vi "VIH UI - Property Page - File.vi"() -> ()   [LabVIEW 2014]
doc: "::: VI Helpeks :::\nCopyright (c) 2000-2026 Konstantin Shifershteyn. All rights reserved."
uses:
  _VIH HelpGen.llb/VIH HelpGen Typedef - Enum - Default,Enable,Disable.ctl
  _VIH HelpGen.llb/VIH HelpGen Typedef - Enum - Description Mode.ctl
  _VIH UI Controls.llb/VIH UI Control - Button - Insert HREF.ctl
  _VIH UI Controls.llb/VIH UI Control - Button - Insert Bold.ctl
  _VIH UI Controls.llb/VIH UI Control - Button - Insert Italic.ctl
  _VIH UI Controls.llb/VIH UI Control - Button - Insert Underline.ctl
  _VIH Project Manager.llb/VIH Project Tree Typedef - Tree Refnum.ctl
  VIH UI Typedef - Property Page ExtCommand.ctl
  <vilib>/Utility/miscctls.llb/LVPositionTypeDef.ctl
  <vilib>/Utility/miscctls.llb/LVPointTypeDef.ctl
  <vilib>/Utility/miscctls.llb/LVRowAndColumnUnsignedTypeDef.ctl
  <vilib>/Utility/miscctls.llb/LVSelectionTypeDef.ctl
  _VIH HelpGen - Palette.llb/VIH HelpGen Typedef - Palette - Item Type Enum.ctl
  _VIH Support Library.llb/VIH Utility - APP - Is Value Changed (STR).vi
  _VIH Support Library.llb/VIH Utility - APP - Is Value Changed (BOOL).vi
panel:
  out "CategoryTitle":string
  in  "%UPDATE":bool
  in  "%STOP":bool
  in  "Category List":i32(listbox)
  in  "TreeRef":T1
  in  "Tab Control":enum32{"0", "1", "2", "3", "4", "5", "6", "7"}(tab) caption="File Rule"
  out "PI_AddInfo":string caption="Additional Information"
  out "PI_Email":string caption="Contact E-mail"
  out "PI_Website":string caption="Website"
  out "PI_Version":string caption="Version"
  out "PI_Copyright":string caption="Legal Copyright"
  out "PI_Company":string caption="Company Name"
  out "PI_Author":string caption="Author Name"
  out "PI_Product":string caption="Product Name"
  in  "ProductInfoText":string caption="Product Info section"
  in  "ProductInfoMode":u16(ring) caption="Product Info mode" items=["Default", "Custom", "Disable"]
  out "Out File Path":path caption="Output File Path"
  in  "Out File Name":string caption="Output File Name"
  in  "Custom_OutFile":i16(ring) caption="Default/Custom selector" items=["Default", "Custom"]
  in  "BuildHelp":T2 caption="Build help for this file"
  out "File Name":string
  in  "Comments":string
  in  "Custom_JS Dir":i16(ring) caption="Default/Custom selector" items=["Default", "Custom"]
  in  "Dst_JS Dir":path caption="Subfolder to save JavaScript files"
  in  "Custom_CSS Dir":i16(ring) caption="Default/Custom selector" items=["Default", "Custom"]
  in  "Dst_CSS Dir":path caption="Subfolder to save CSS files"
  in  "Custom_Image Dir":i16(ring) caption="Default/Custom selector" items=["Default", "Custom"]
  in  "Dst_Image Dir":path caption="Subfolder to save image files"
  in  "Custom_HTML Dir":i16(ring) caption="Default/Custom selector" items=["Default", "Custom"]
  in  "Dst_HTML Dir":path caption="Subfolder to save HTML files"
  out "Build Root Dir":path caption="Build Root Folder"
  in  "Src_Template":path caption="Help Template File"
  in  "Custom_Template":i16(ring) caption="Default/Custom selector" items=["Default", "Custom"]
  out "JS File":path caption="JS File Path"
  in  "JS List":i32[](listbox) caption="JavaScript Files"
  in  "%JS List_Add":bool caption="Add JavaScript File"
  in  "%JS List_Remove":bool caption="Remove JavaScript File"
  in  "Override_JS Files":bool caption="Override default JS file set"
  out "CSS File":path caption="CSS File Path"
  in  "CSS List":i32[](listbox) caption="CSS Files"
  in  "%CSS List_Add":bool caption="Add CSS File"
  in  "%CSS List_Remove":bool caption="Remove CSS File"
  in  "Override_CSS Files":bool caption="Override default CSS file set"
  in  "%VIDetails_Insert_<I>":T3 caption="Format as Italic"
  in  "%VIDetails_Insert_<U>":T4 caption="Format as Underline"
  in  "%VIDetails_Insert_<B>":T5 caption="Format as Bold"
  in  "%VIDetails_Insert_HREF":T6 caption="Insert Reference"
  in  "VIDetails":string caption="Details section"
  in  "VIDetailsMode":T7 caption="Details section mode"
  in  "%VIDscr_Insert_<I>":T3 caption="Format as Italic"
  in  "%VIDscr_Insert_<U>":T4 caption="Format as Underline"
  in  "%VIDscr_Insert_<B>":T5 caption="Format as Bold"
  in  "%VIDscr_Insert_HREF":T6 caption="Insert Reference"
  in  "VIDescription":string caption="Description"
  in  "MenuItemIcons":T2 caption="Generate Palette Item Icons"
  in  "VIDscrMode":T7 caption="Description mode"
  in  "Ctl_EnumValues":T2 caption="Build list of Enum and Ring values"
  in  "Ctl_ClustMembers":T2 caption="Expand cluster members"
  in  "Ctl_DscrMode":T7 caption="VI Controls/Terminals description mode"
  in  "%CtrlRule_Insert_<I>":T3 caption="Format as Italic"
  in  "%CtrlRule_Insert_<U>":T4 caption="Format as Underline"
  in  "%CtrlRule_Insert_<B>":T5 caption="Format as Bold"
  in  "%CtrlRule_Insert_HREF":T6 caption="Insert Reference"
  in  "CtrlRule_Description":string caption="Description"
  in  "CtrlRule_CustomName":string caption="Custom Control Name"
  in  "CtrlRule_DscrMode":T7 caption="Description mode"
  in  "CtrlRule_CustomRule":bool caption="Enable custom rule"
  in  "CtrlRule_CtrlID":string caption="Control Identifier"
  in  "%CtrlRule_Edit_Enum":bool caption="Edit Enumerated Values Description"
  in  "CtrlRule_EnumValues":T2 caption="Enum and Ring values"
  in  "CtrlRule_ClustMembers":T2 caption="Cluster members"
  in  "%CtrlRule_Copy":bool caption="Copy"
  in  "%CtrlRule_Paste":bool caption="Paste"
  in  "%CtrlRule_Import":bool caption="Import VI Terminal Controls"
  in  "CtrlRule List":i32[](listbox) caption="Control List"
  in  "%CtrlRule_Remove":bool caption="Remove"
  in  "%CtrlRule_Add":bool caption="Add"
  in  "Override_Ctl Rules":bool caption="Override default Control Rules definition"
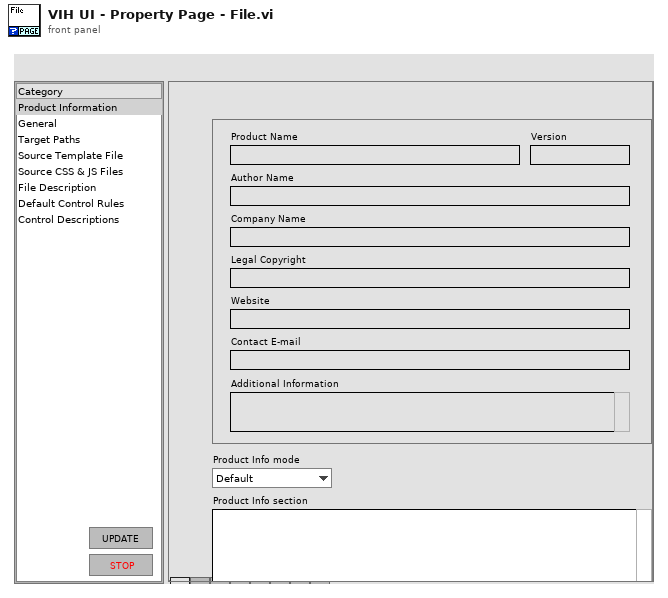
[diagram p1: front panel]
types:
  T1 = typedef "VIH Project Tree Typedef - Tree Refnum.ctl" = refnum<vi>
  T2 = typedef "VIH HelpGen Typedef - Enum - Default,Enable,Disable.ctl" = enum16{"Default", "Enable", "Disable"}
  T3 = typedef "VIH UI Control - Button - Insert Italic.ctl" = bool
  T4 = typedef "VIH UI Control - Button - Insert Underline.ctl" = bool
  T5 = typedef "VIH UI Control - Button - Insert Bold.ctl" = bool
  T6 = typedef "VIH UI Control - Button - Insert HREF.ctl" = bool
  T7 = typedef "VIH HelpGen Typedef - Enum - Description Mode.ctl" = enum16{"Default", "Description", "Description1", "Description2", "Custom", "None"}
  T8 = typedef "VIH UI Typedef - Property Page ExtCommand.ctl" = cluster{"Action":string, "Project Tree":T1, "Params":string[]}
  T9 = enum16{"Open", "Close", "Update", "Set Category"}
  T10 = enum32{"Invalid", "Standard", "Closed", "Hidden", "Minimized", "Maximized"}
  T11 = enum8{"Enabled", "Disabled", "Disabled and Grayed Out"}
  T12 = typedef "LVSelectionTypeDef.ctl" = cluster{"Selection Start":u32, "Selection End":u32}
  T13 = enum16{"get", "get all", "set", "Init", "delete", "rename"}
  T14 = typedef "eventvkey.ctl" = enum16{"ASCII", "Enter", "Return", "Shift", "Ctrl", "Alt", "Cmd", "Opt", "Caps", "NumLock", "Clear", "Break", "Up", "Down", "Left", "Right", "Insert", "Delete", "Home", "End", "PageUp", "PageDown", "Escape", "Help", "Pause", "ScrollLock", "F1", "F2", "F3", "F4", "F5", "F6", "F7", "F8", "F9", "F10", "F11", "F12", "F13", "F14", "F15", "F16", "F17", "F18", "F19", "F20", "F21", "F22", "F23", "F24", "Play", "VolumeUp", "VolumeDown", "Mute", "Two Byte Char"}
  T15 = cluster{"Shift":bool, "Ctrl":bool, "Alt":bool, "Cmd":bool, "Opt":bool}
  T16 = typedef "VIH HelpGen Typedef - Cluster - Group Rule.ctl" = cluster{"Source Root Dir":path, "Build Root Dir":path, "BuildHelp":T2, "Source Paths":T17, "Target Paths":T18, "VIDscrMode":T7, "MenuDscrMode":T7, "MenuItemIcons":T2, "Control Rules":T19[], "Flags":T21, "Ctl_DscrMode":T7, "Ctl_ClustMembers":T2, "Ctl_EnumValues":T2, "%Comments":string, "PVIIDscrMode":T7, "VIDetailsMode":T7, "ProductInfoMode":T2, "ProductInfoText":string}
  T17 = typedef "VIH HelpGen Typedef - Cluster - Group Rule - Source Paths.ctl" = cluster{"CSS Files":path[], "JS Files":path[], "VI Template":path, "Menu Template":path, "PolyVI Template":path}
  T18 = typedef "VIH HelpGen Typedef - Cluster - Group Rule - Target Paths.ctl" = cluster{"HTML Dir":path, "Image Dir":path, "CSS Dir":path, "JS Dir":path}
  T19 = typedef "VIH HelpGen Typedef - Cluster - Control Rule.ctl" = cluster{"CtrlID":string, "CustomRule":bool, "DscrMode":T7, "Description":string, "ClusterMembers":T2, "EnumValues":T2, "EnumValDscr":T20[], "CustomName":string}
  T20 = typedef "VIH HelpGen Typedef - Cluster - Enum Value Info.ctl" = cluster{"Value":ext, "String":string, "Description":string}
  T21 = typedef "VIH HelpGen Typedef - Cluster - Group Rule - Flags.ctl" = cluster{"Override CSS Files":bool, "Override JS Files":bool, "Override Ctl Rules":bool}
  T22 = typedef "LVPoint32TypeDef.ctl" = cluster{"Horizontal":i32, "Vertical":i32}
  T23 = typedef "LVRowAndColumnTypeDef.ctl" = cluster{"Row":i32, "Column":i32}
  T24 = typedef "lveventtype.ctl" = enum32{"Null", "Timeout", "Annotation Menu Selection", "Annotation Menu Selection?", "App Instance Close", "App Instance Close?", "Autoscale Range Change", "Bookmark Info Change", "Cell Edit", "Cell Edit?", "Cursor Grab", "Cursor Grab?", "Cursor Menu Selection", "Cursor Menu Selection?", "Cursor Move", "Cursor Release", "Data Change", "Direction Change", "Display State Change", "Drag Ended", "Drag Enter", "Drag Leave", "Drag Over", "Drag Source Update", "Drag Starting", "Drag Starting?", "Drop", "Exec State Change", "Key Down", "Key Down?", "Key Repeat", "Key Repeat?", "Key Up", "Listbox Double Click", "Menu Activation?", "Menu Selection (App)", "Menu Selection? (App)", "Menu Selection (User)", "Mouse Down", "Mouse Down?", "Mouse Enter", "Mouse Leave", "Mouse Move", "Mouse Up", "Mouse Wheel", "NI Security User Change (App)", "Pane Size", "Panel Close", "Panel Close?", "Panel Resize", "Plot Attribute Change", "Scale Range Change", "Shortcut Menu Activation?", "Shortcut Menu Selection (App)", "Shortcut Menu Selection? (App)", "Shortcut Menu Selection (User)", "Tree Double Click", "Tree Drag", "Tree Drag?", "Tree Drop", "Tree Drop?", "Tree Item Close", "Tree Item Close?", "Tree Item Open", "Tree Item Open?", "User Event", "Value Change"}
  T25 = typedef "LVPointTypeDef.ctl" = cluster{"Horizontal":i16, "Vertical":i16}
  T26 = typedef "LVPositionTypeDef.ctl" = cluster{"Left":i32, "Top":i32}
  T27 = typedef "LVRowAndColumnUnsignedTypeDef.ctl" = cluster{"Row":u32, "Column":u32}
  T28 = typedef "VIH Project Tree Typedef - Tree Item Type.ctl" = enum32{"<Invalid>", "Project", "Proj Files", "Proj Rules", "File Group", "Rule Group", "Any File", "LV Func", ".mnu", ".mnu (dyn)", ".vi", ".vi (dyn)", ".vit", ".vit (dyn)", ".ctl", ".ctl (dyn)", ".ctt", ".ctt (dyn)", "polyVI", "polyVI (dyn)", "expVI", "expVI (dyn)", "HTML", "PolyVI Inst"}
  T29 = typedef "VIH HelpGen Typedef - Cluster - File Rule.ctl" = cluster{"OutName":string, "BuildHelp":T2, "Source Paths":T30, "Target Paths":T31, "DscrMode":T7, "Description":string, "Control Rules":T19[], "Flags":T21, "Ctl_DscrMode":T7, "Ctl_ClustMembers":T2, "Ctl_EnumValues":T2, "MenuItemIcons":T2, "%Comments":string, "DetailsMode":T7, "DetailsText":string, "ProductInfoMode":T2, "ProductInfoText":string}
  T30 = typedef "VIH HelpGen Typedef - Cluster - File Rule - Source Paths.ctl" = cluster{"CSS Files":path[], "JS Files":path[], "Html Template":path}
  T31 = typedef "VIH HelpGen Typedef - Cluster - File Rule - Target Paths.ctl" = cluster{"HTML Dir":path, "Image Dir":path, "CSS Dir":path, "JS Dir":path}
  T32 = cluster{"Array out":string[], "Item Rule out":T29}
  T33 = typedef "VIH HelpGen Typedef - Palette - Item Type Enum.ctl" = enum32{"<Invalid>", "<unknown>", "VI", "Menu", "LV Func", "Express VI", "Poly VI", "CTL", "HTML"}
  T34 = typedef "VIH HelpGen Typedef - Product Info Cluster.ctl" = cluster{"ProductName":string, "Version":string, "Author":string, "Company":string, "Copyright":string, "Website":string, "Email":string, "AddInfo":string}
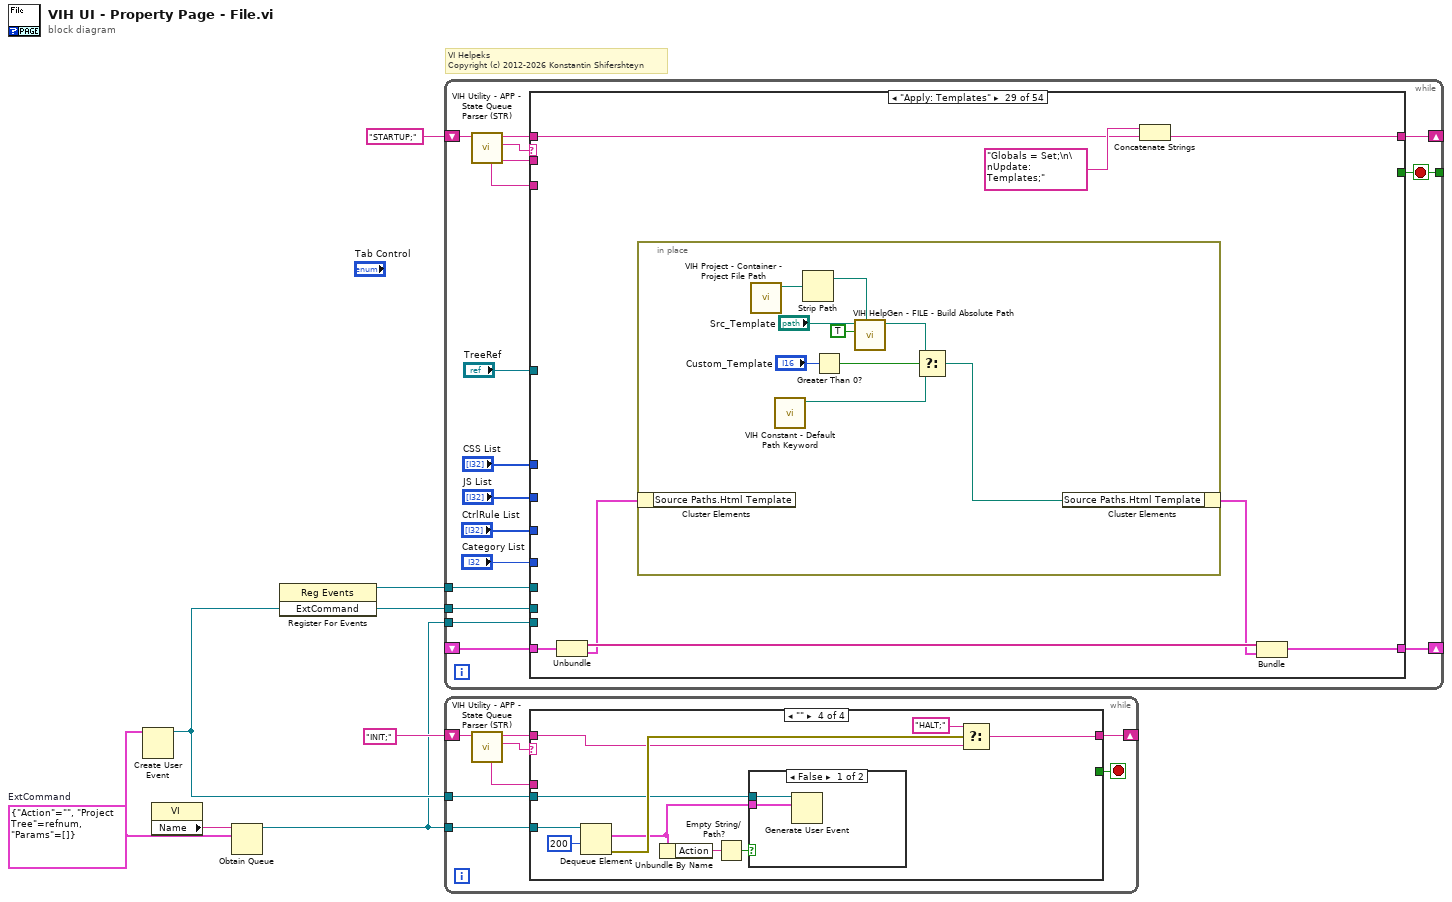
[diagram p0: block diagram]
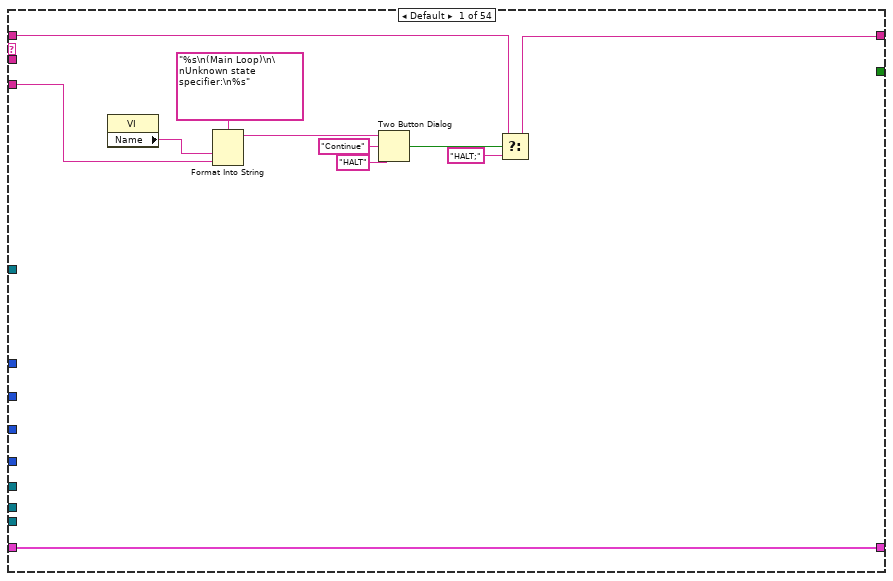
[diagram p2: hidden frame]
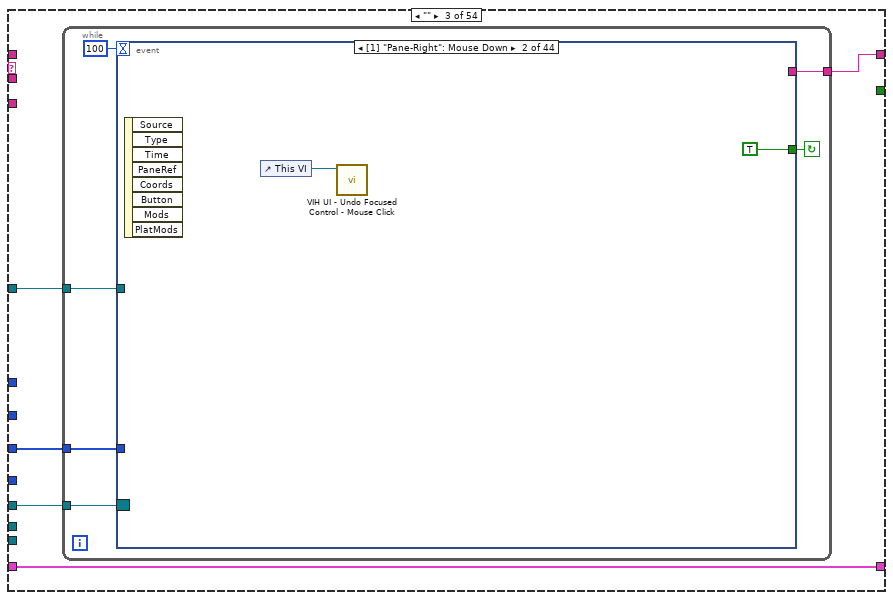
[diagram p4: hidden frame]
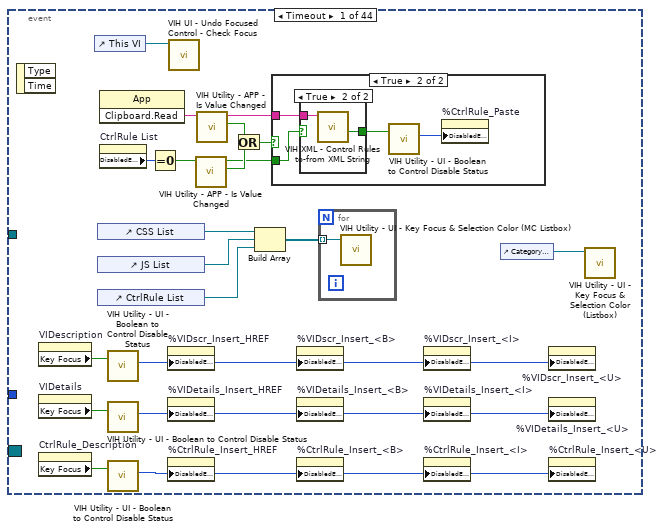
[diagram p5: hidden frame]
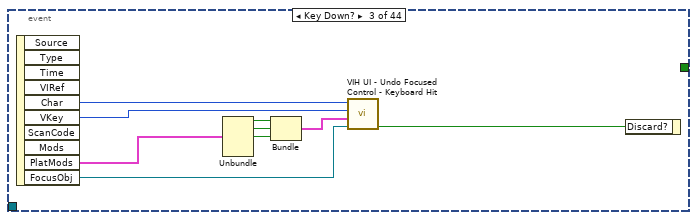
[diagram p8: hidden frame]
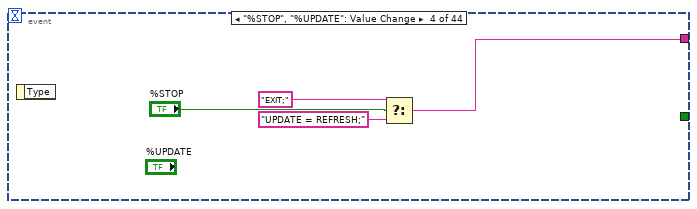
[diagram p9: hidden frame]
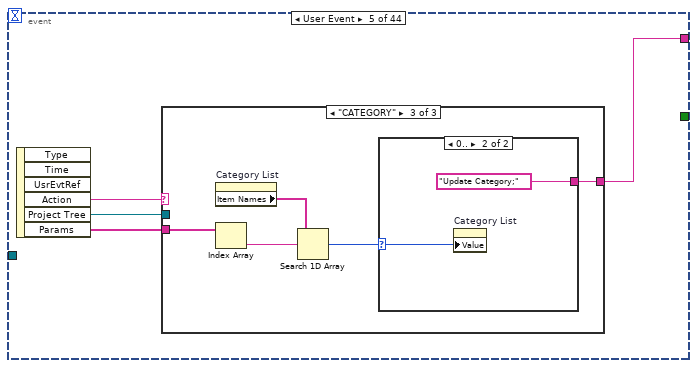
[diagram p10: hidden frame]
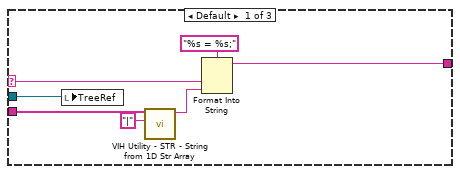
[diagram p11: hidden frame]
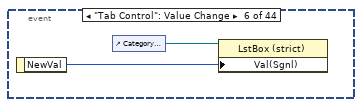
[diagram p14: hidden frame]
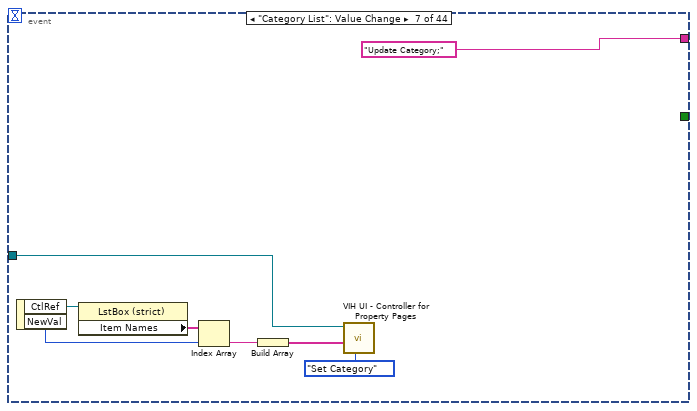
[diagram p15: hidden frame]
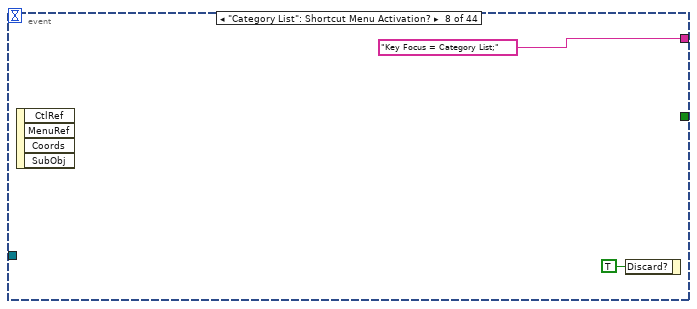
[diagram p16: hidden frame]
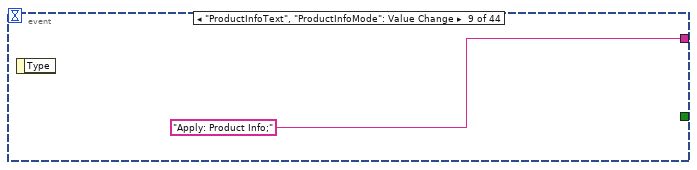
[diagram p17: hidden frame]
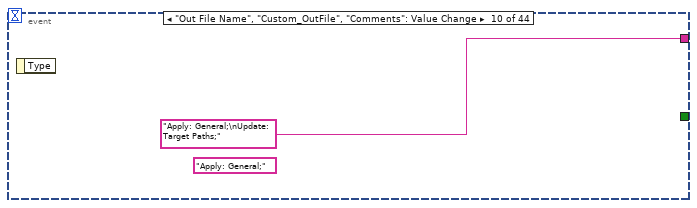
[diagram p18: hidden frame]
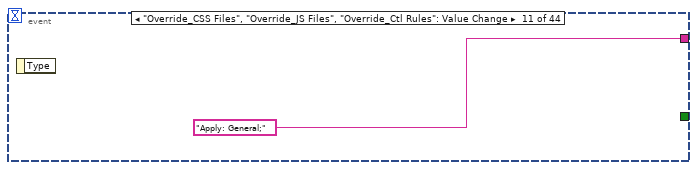
[diagram p19: hidden frame]
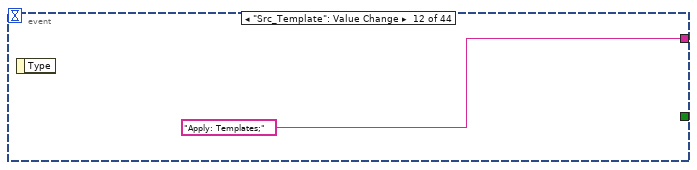
[diagram p20: hidden frame]
diagram:
  w1 = T8 {"Action"="", "Project Tree"=refnum, "Params"=[]}  # ExtCommand
  # "VI Helpeks\nCopyright (c) 2012-2026 Konstantin Shifershteyn"
  n1 = Create User Event(user event datatype=w1) -> (user event=w3:refnum<user-event>)  [unwired: 1 in, 1 out]
  n2 = property class="VI"() -> ("Name"=w6:string)  [unwired: 2 in, 2 out]
  n3 = Obtain Queue(name (unnamed)=w6, element data type=w1) -> (queue out=w2:refnum<queue>)  [unwired: 3 in, 2 out]
  n4 = register-events(w3) -> (reference out=w5:refnum<event-registration>)  [unwired: 2 in, 1 out]
  n5 = while {
    shift-right: [w21] -> _
    shift-left: "STARTUP;" -> [w24]
    tunnel: [w19] -> _
    tunnel: w5 -> [w18]
    tunnel: w3 -> [w17]
    tunnel: w2 -> [w16]
    shift-right: [w13] -> _
    shift-left: _ -> [w12]
    stop <- w19 stop-if-true
    n6 = call "VIH Utility - APP - State Queue Parser (STR).vi"("input queue"=w24) -> ("state parameters"=w15:string, "state"=w23:string, "remained queue"=w20:string, "complete state specifier"=w22:string)  [unwired: 5 in]
    n7 = case shown="\"Apply: Templates\"" w23 {
      tunnel: w22 -> [w31 _ _ _ _ _ _ _ _ w469 _ _ _ _ _ _ _ _ _ _ _ _ _ _ _ _ _ _ _ _ _ _ _ _ _ _ _ _ _ _ _ _ _ _ _ _ _ _ _ _ _ _ _ _]
      tunnel: [w26 w36 w41 "INIT;\nUPDATE;" w391 "HALT;" w417 w420 w444 w471 w497 w521 w525 w541 w547 w557 w620 w693 w716 w772 w803 w815 w878 w901 w921 w922 w935 w954 w979 w996 w1013 w1030 w1077 w1105 w1148 w1155 w1179 w1195 w1231 w1253 w1280 w1288 w1306 w1318 w1344 w1368 w1383 w1391 w1409 w1421 w1447 w1471 w1486 w1488] -> w21
      tunnel: w20 -> [w27 w36 _ _ w391 _ w417 w420 w445 w471 w497 w521 w525 w541 w547 w557 w620 w693 w716 w772 w803 w843 w878 w901 w921 w923 w941 w955 w980 w997 w1013 w1030 w1082 w1106 w1148 w1160 w1184 w1202 w1236 w1260 w1280 w1288 w1306 w1322 w1349 w1373 w1383 w1391 w1409 w1425 w1452 w1476 w1486 w1488]
      tunnel: [_ _ _ _ _ _ TRUE _ _ _ _ _ _ _ _ _ _ _ _ _ _ _ _ _ _ _ _ _ _ _ _ _ _ _ _ _ _ _ _ _ _ _ _ _ _ _ _ _ _ _ _ _ _ _] -> w19
      tunnel: w18 -> [_ _ w42 _ _ _ w416 _ _ _ _ _ _ _ _ _ _ _ _ _ _ _ _ _ _ _ _ _ _ _ _ _ _ _ _ _ _ _ _ _ _ _ _ _ _ _ _ _ _ _ _ _ _ _]
      tunnel: w17 -> [_ _ _ _ _ _ w415 _ _ _ _ _ _ _ _ _ _ _ _ _ _ _ _ _ _ _ _ _ _ _ _ _ _ _ _ _ _ _ _ _ _ _ _ _ _ _ _ _ _ _ _ _ _ _]
      tunnel: w16 -> [_ _ _ _ _ _ w413 _ _ _ _ _ _ _ _ _ _ _ _ _ _ _ _ _ _ _ _ _ _ _ _ _ _ _ _ _ _ _ _ _ _ _ _ _ _ _ _ _ _ _ _ _ _ _]
      tunnel: w15 -> [_ _ _ _ _ _ _ _ w431 w470 _ w519 w523 _ _ _ _ _ _ w761 w794 _ _ w888 _ _ _ _ _ _ _ w1014 _ w1100 _ _ _ w1193 w1228 w1251 _ _ _ _ _ _ _ _ _ _ _ _ _ _]
      tunnel: "Category List" -> [_ _ _ _ _ _ _ _ _ _ w494 _ _ _ _ _ _ _ _ _ _ _ _ _ _ _ _ _ _ _ _ _ _ _ _ _ _ _ _ _ _ _ _ _ _ _ _ _ _ _ _ _ _ _]
      tunnel: [w25 w37 w40 w363 w390 w398 w411 w419 w442 w473 w491 w520 w524 w540 w546 w574 w619 w692 w715 w771 w802 w842 w877 w900 w920 w927 w938 w959 w984 w1001 w1012 w1029 w1078 w1104 w1145 w1156 w1180 w1197 w1232 w1255 w1279 w1286 w1305 w1319 w1345 w1369 w1382 w1389 w1408 w1422 w1448 w1472 w1485 w1487] -> w13
      tunnel: w12 -> [w25 w37 w40 w363 w390 w398 w411 w419 w441 w472 w491 w520 w524 w540 w546 w574 w619 w692 w715 w771 w802 w842 w877 w900 w920 w929 w940 w961 w986 w1003 w1012 w1029 w1079 w1095 w1145 w1157 w1181 w1198 w1233 w1256 w1279 w1286 w1305 w1320 w1346 w1370 w1382 w1389 w1408 w1423 w1449 w1473 w1485 w1487]
      tunnel: "CtrlRule List" -> [_ _ w39 _ _ _ _ _ _ _ _ _ _ _ _ _ _ _ _ _ _ _ _ w890 _ _ _ _ _ _ _ w1021 w1071 w1098 w1146 w1153 _ _ _ _ _ _ _ _ _ _ _ _ _ _ _ _ _ _]
      tunnel: "CSS List" -> [_ _ _ _ _ _ _ _ _ _ _ _ _ _ _ _ _ _ _ w763 _ _ _ _ _ _ _ _ _ _ _ _ _ _ _ _ _ _ _ _ _ w1285 _ w1310 w1342 _ _ _ _ _ _ _ _ _]
      tunnel: "JS List" -> [_ _ _ _ _ _ _ _ _ _ _ _ _ _ _ _ _ _ _ _ w793 _ _ _ _ _ _ _ _ _ _ _ _ _ _ _ _ _ _ _ _ _ _ _ _ _ _ w1387 _ w1411 w1445 _ _ _]
      tunnel: "TreeRef" -> [_ _ w38 _ _ _ _ _ _ _ _ _ _ _ _ _ _ w656 w707 _ _ _ _ _ _ _ _ _ _ _ _ _ _ w1096 _ _ _ _ _ w1250 _ _ _ _ _ _ _ _ _ _ _ _ _ _]
      frame Default {
        n8 = property class="VI"() -> ("Name"=w30:string)  [unwired: 2 in, 2 out]
        n9 = Format Into String(format string="%s\n(Main Loop)\n\nUnknown state specifier:\n%s", w30, w31) -> (resulting string=w34:string)  [unwired: 2 in, 1 out]
        n10 = Two Button Dialog(message=w34, 1:"HALT" ("F button name (\"Cancel\")"), 2:"Continue" ("T button name (\"OK\")")) -> (T button?=w28:bool)
        n11 = Select(t=w27, s=w28, f="HALT;") -> (s? t:f=w26:string)
      }
      frame "#" {
      }
      frame "" {
        n12 = while {
          tunnel: w42 -> [w47]
          tunnel: [w46] -> w41
          tunnel: w39 -> [w45]
          tunnel: w38 -> [w44]
          stop <- w43 continue-if-true
          n13 = event shown="[1] \"Pane-Right\": Mouse Down" {
            selector: w47 -> [_ _ _ _ _ _ _ _ _ _ _ _ _ _ _ _ _ _ _ _ _ _ _ _ _ _ _ _ _ _ _ _ _ _ _ _ _ _ _ _ _ _ _ _]
            dyn-events: _ -> [_ _ _ _ _ _ _ _ _ _ _ _ _ _ _ _ _ _ _ _ _ _ _ _ _ _ _ _ _ _ _ _ _ _ _ _ _ _ _ _ _ _ _ _]
            timeout: 100 -> [_ _ _ _ _ _ _ _ _ _ _ _ _ _ _ _ _ _ _ _ _ _ _ _ _ _ _ _ _ _ _ _ _ _ _ _ _ _ _ _ _ _ _ _]
            tunnel: [_ _ _ w89 w95 _ "Update Category;" ("string") "Key Focus = Category List;" ("output string") "Apply: Product Info;" ("string") "Apply: General;\nUpdate: Target Paths;" ("string") "Apply: General;" ("string") "Apply: Templates;" ("string") "Apply: Templates;" ("string") "Apply: Target Paths;" ("string") "Apply: Target Paths;" ("string") "Apply: Item Rules;" ("string") "Apply: Item Rules;" ("string") "CtrlRule: Update Controls = INIT;" ("string") w171 w185 w200 w215 "Key Focus = CtrlRule List;" ("output string") w219 w229 w242 w248 "CSS List: Update Controls;" w254 "Key Focus = CSS List;" ("output string") w258 "JS List: Update Controls;" w267 "Key Focus = JS List;" ("output string") w271 _ _ _ _ _ _ _ _ _] -> w46
            tunnel: w45 -> [_ _ _ _ _ _ _ _ _ _ _ _ _ _ _ _ _ _ _ w183 _ _ _ _ _ w235 w245 _ _ _ _ _ _ _ _ _ _ _ _ _ _ _ _ _]
            tunnel: w44 -> [_ _ _ _ _ _ w112 _ _ _ _ _ _ _ _ _ _ _ _ _ _ _ _ _ _ _ _ _ _ _ _ _ _ _ _ w284 w297 w309 w318 w322 w327 w331 w336 w340]
            tunnel: [_ TRUE _ _ _ _ _ _ _ _ _ _ _ _ _ _ _ _ _ _ _ _ _ _ _ _ _ _ _ _ _ _ _ _ _ _ _ _ _ _ _ _ _ _] -> w43
            event Timeout {
              n14 = event-data() -> ()  [unwired: 1 in, 2 out]
              n15 = property on="VIDescription" class="Str"() -> ("Key Focus"=w59:bool)  [unwired: 2 in, 2 out]
              n16 = property on="VIDetails" class="Str"() -> ("Key Focus"=w51:bool)  [unwired: 2 in, 2 out]
              n17 = property on="CtrlRule_Description" class="Str"() -> ("Key Focus"=w61:bool)  [unwired: 2 in, 2 out]
              n18 = control-ref of="This VI"() -> (w49:refnum<vi>)
              n19 = control-ref of="CSS List"() -> (w66:refnum<vi>)
              n20 = control-ref of="JS List"() -> (w65:refnum<vi>)
              n21 = control-ref of="CtrlRule List"() -> (w64:refnum<vi>)
              n22 = invoke class="App" method="Clipboard.Read"() -> ("Read Clipbrd"=w63:string)  [unwired: 3 in, 2 out]
              n23 = property on="CtrlRule List" class="MCListbox (strict)"() -> ("DisabledEnum"=w57:T11)  [unwired: 2 in, 2 out]
              n24 = call "VIH Utility - UI - Boolean to Control Disable Status.vi"("Status in"=w59) -> ("Control Disable if False"=w58:u8)  [unwired: 3 in, 1 out]
              n25 = call "VIH Utility - UI - Boolean to Control Disable Status.vi"("Status in"=w51) -> ("Control Disable if False"=w50:u8)  [unwired: 3 in, 1 out]
              n26 = call "VIH Utility - UI - Boolean to Control Disable Status.vi"("Status in"=w61) -> ("Control Disable if False"=w60:u8)  [unwired: 3 in, 1 out]
              n27 = Equal To 0?(x=w57) -> (x = 0?=w56:bool)
              n28 = property on="%VIDscr_Insert_HREF" class="Bool"("DisabledEnum"=w58) -> ()  [unwired: 2 in, 2 out]
              n29 = property on="%VIDetails_Insert_HREF" class="Bool"("DisabledEnum"=w50) -> ()  [unwired: 2 in, 2 out]
              n30 = property on="%CtrlRule_Insert_HREF" class="Bool"("DisabledEnum"=w60) -> ()  [unwired: 2 in, 2 out]
              n31 = call "VIH UI - Undo Focused Control - Check Focus.vi"("VI Refnum"=w49) -> ()  [unwired: 10 in, 1 out]
              n32 = call-poly "VIH Utility - APP - Is Value Changed.vi"("Value"=w56) -> ("Changed"=w54:bool, "dup Value"=w52:bool)  [unwired: 5 in]
              n33 = call-poly "VIH Utility - APP - Is Value Changed.vi"("Value"=w63) -> ("Changed"=w55:bool, "dup Value"=w62:string)  [unwired: 5 in]
              n34 = Or(x=w55, y=w54) -> (x .or. y?=w53:bool)
              n35 = Build Array(w66, w65, w64) -> (w68:refnum<vi>[])
              n36 = case shown="True" w53 {
                tunnel: w62 -> [_ w70]
                tunnel: w52 -> [_ w69]
                frame False {
                }
                frame True {
                  n37 = case shown="True" w69 {
                    selector: w69 -> [w73 _]
                    tunnel: [w73 w75] -> w72
                    tunnel: w70 -> [_ w74]
                    frame False {
                    }
                    frame True {
                      n38 = call "VIH XML - Control Rules to-from XML String.vi"("XML in"=w74) -> ("available"=w75:bool)  [unwired: 7 in, 3 out]
                    }
                  }
                  n39 = call "VIH Utility - UI - Boolean to Control Disable Status.vi"("Status in"=w72) -> ("Control Disable if False"=w71:u8)  [unwired: 3 in, 1 out]
                  n40 = property on="%CtrlRule_Paste" class="Bool"("DisabledEnum"=w71) -> ()  [unwired: 2 in, 2 out]
                }
              }
              n41 = property on="%VIDscr_Insert_<B>" class="Bool"("DisabledEnum"=w58) -> ()  [unwired: 2 in, 2 out]
              n42 = property on="%VIDetails_Insert_<B>" class="Bool"("DisabledEnum"=w50) -> ()  [unwired: 2 in, 2 out]
              n43 = property on="%CtrlRule_Insert_<B>" class="Bool"("DisabledEnum"=w60) -> ()  [unwired: 2 in, 2 out]
              n44 = for {
                tunnel: w68 -> [w76] mode=indexing
                n45 = call "VIH Utility - UI - Key Focus & Selection Color (MC Listbox).vi"("MCListbox Refnum"=w76) -> ()  [unwired: 8 in, 3 out]
              }
              n46 = property on="%VIDscr_Insert_<I>" class="Bool"("DisabledEnum"=w58) -> ()  [unwired: 2 in, 2 out]
              n47 = property on="%VIDetails_Insert_<I>" class="Bool"("DisabledEnum"=w50) -> ()  [unwired: 2 in, 2 out]
              n48 = property on="%CtrlRule_Insert_<I>" class="Bool"("DisabledEnum"=w60) -> ()  [unwired: 2 in, 2 out]
              n49 = control-ref of="Category List"() -> (w67:refnum<vi>)
              n50 = property on="%VIDscr_Insert_<U>" class="Bool"("DisabledEnum"=w58) -> ()  [unwired: 2 in, 2 out]
              n51 = property on="%VIDetails_Insert_<U>" class="Bool"("DisabledEnum"=w50) -> ()  [unwired: 2 in, 2 out]
              n52 = property on="%CtrlRule_Insert_<U>" class="Bool"("DisabledEnum"=w60) -> ()  [unwired: 2 in, 2 out]
              n53 = call "VIH Utility - UI - Key Focus & Selection Color (Listbox).vi"("LstBox Refnum"=w67) -> ()  [unwired: 8 in, 3 out]
            }
            event Mouse Down {
              n54 = event-data() -> ()  [unwired: 1 in, 8 out]
              n55 = control-ref of="This VI"() -> (w78:refnum<vi>)
              n56 = call "VIH UI - Undo Focused Control - Mouse Click.vi"("VI Refnum"=w78) -> ()  [unwired: 9 in, 2 out]
            }
            event Key Down? {
              n57 = event-data() -> ("Char"=w83:i16, "VKey"=w82:T14, "PlatMods"=w81:T15, "FocusObj"=w80:refnum<vi>)  [unwired: 1 in, 6 out]
              n58 = Unbundle(w81) -> ("Shift"=w84:bool, "Ctrl"=w85:bool, "Alt"=w86:bool)  [unwired: 2 out]
              n59 = Bundle("Shift"=w84, "Ctrl"=w85, "Alt"=w86) -> (w87:cluster{"Shift":bool, "Ctrl":bool, "Alt":bool})  [unwired: 1 in]
              n60 = call "VIH UI - Undo Focused Control - Keyboard Hit.vi"("FocusObj"=w80, "PlatMods"=w87, "VKey"=w82, "Char"=w83) -> ("Discard"=w79:bool)  [unwired: 7 in]
              n61 = event-data("Discard?"=w79) -> ()  [unwired: 1 in, 1 out]
            }
            event "%STOP", "%UPDATE": Value Change {
              n62 = event-data() -> ()  [unwired: 1 in, 1 out]
              n63 = Select(t="EXIT;", s="%STOP", f="UPDATE = REFRESH;") -> (s? t:f=w89:string)
            }
            event User Event {
              n64 = event-data() -> ("Action"=w93:string, "Project Tree"=w92:T1, "Params"=w94:string[])  [unwired: 1 in, 3 out]
              n65 = case shown="\"CATEGORY\"" w93 {
                selector: w93 -> [w97 _ _]
                tunnel: w94 -> [w102 _ w107]
                tunnel: [w98 _ w103] -> w95
                tunnel: w92 -> [w96 _ _]
                frame Default {
                  n66 = local write "TreeRef"(w96) -> ()
                  n67 = call "VIH Utility - STR - String from 1D Str Array.vi"("delimiter ('\\n')"="|" ("delimiter ('\\n')"), "Array in"=w102) -> ("String out"=w99:string)  [unwired: 5 in]
                  n68 = Format Into String(format string="%s = %s;", w97, w99) -> (resulting string=w98:string)  [unwired: 2 in, 1 out]
                }
                frame "" {
                }
                frame "CATEGORY" {
                  n69 = property on="Category List" class="LstBox (strict)"() -> ("Item Names"=w105:string[])  [unwired: 2 in, 2 out]
                  n70 = Index Array(array=w107) -> (element=w106:string)  [unwired: 1 in]
                  n71 = Search 1D Array(1D array=w105, element=w106) -> (index of element=w104:i32)  [unwired: 1 in]
                  n72 = case shown="0.." w104 {
                    selector: w104 -> [_ w109]
                    tunnel: [_ "Update Category;" ("string")] -> w103
                    frame ..-1 {
                    }
                    frame 0.. {
                      n73 = property on="Category List" class="LstBox (strict)"("Value"=w109) -> ()  [unwired: 2 in, 2 out]
                    }
                  }
                }
              }
            }
            event "Tab Control": Value Change {
              n74 = event-data() -> ("NewVal"=w110:enum32{"0", "1", "2", "3", "4", "5", "6", "7"})  [unwired: 1 in]
              n75 = control-ref of="Category List"() -> (w111:refnum<vi>)
              n76 = property class="LstBox (strict)"(reference=w111, "Val(Sgnl)"=w110) -> ()  [unwired: 1 in, 2 out]
            }
            event "Category List": Value Change {
              n77 = event-data() -> ("CtlRef"=w118:refnum<vi>, "NewVal"=w116:i32)  [unwired: 1 in]
              n78 = property class="LstBox (strict)"(reference=w118) -> ("Item Names"=w117:string[])  [unwired: 1 in, 2 out]
              n79 = Index Array(array=w117, index=w116) -> (element=w113:string)
              n80 = Build Array(w113) -> (w115:string[])
              n81 = call "VIH UI - Controller for Property Pages.vi"("cmd (update)"=T9."Set Category", "Params"=w115, "Project Tree"=w112) -> ()  [unwired: 7 in, 2 out]
            }
            event "Category List": Shortcut Menu Activation? {
              n82 = event-data() -> ()  [unwired: 1 in, 4 out]
              n83 = event-data("Discard?"=TRUE) -> ()  [unwired: 1 in, 1 out]
            }
            event "ProductInfoText", "ProductInfoMode": Value Change {
              n84 = event-data() -> ()  [unwired: 1 in, 1 out]
            }
            event "Out File Name", "Custom_OutFile", "Comments": Value Change {
              (unwired) "Apply: General;" ("string")
              n85 = event-data() -> ()  [unwired: 1 in, 1 out]
            }
            event "Override_CSS Files", "Override_JS Files", "Override_Ctl Rules": Value Change {
              n86 = event-data() -> ()  [unwired: 1 in, 1 out]
            }
            event "Src_Template": Value Change {
              n87 = event-data() -> ()  [unwired: 1 in, 1 out]
            }
            event "Custom_Template": Value Change {
              n88 = event-data() -> ()  [unwired: 1 in, 1 out]
            }
            event "Dst_HTML Dir", "Dst_Image Dir", "Dst_CSS Dir", "Dst_JS Dir": Value Change {
              n89 = event-data() -> ("CtlRef"=w129:refnum<vi>, "NewVal"=w127:path)  [unwired: 1 in]
              n90 = Empty String/Path?(string/path=w127) -> (empty?=w128:bool)
              n91 = case shown="False" w128 {
                tunnel: w129 -> [w133 _]
                tunnel: w127 -> [w131 _]
                frame False {
                  n92 = Path Type(1:w131) -> (0:w132:i16)
                  n93 = case shown="0" w132 {
                    tunnel: w133 -> [w138 _ w140]
                    tunnel: w131 -> [w135 _ _]
                    frame 0 {
                      # "If absolute path was enered"
                      n94 = call "VIH Project - Container - Master Rule.vi"() -> ("Rule out"=w137:T16)  [unwired: 11 in]
                      n95 = Unbundle By Name(w137) -> ("Build Root Dir"=w134:path)
                      n96 = call "VIH HelpGen - FILE - Build Relative Path.vi"("Root Path"=w134, "Path in"=w135) -> ("Path out"=w136:path)  [unwired: 9 in]
                      n97 = property class="Path"(reference=w138, "Value"=w136) -> ()  [unwired: 1 in, 2 out]
                    }
                    frame 1 {
                    }
                    frame 2, Default {
                      # "Not A Path"
                      n98 = property class="Path"(reference=w140, "Value"=path "") -> ()  [unwired: 1 in, 2 out]
                    }
                  }
                }
                frame True {
                }
              }
            }
            event "Custom_HTML Dir", "Custom_Image Dir", "Custom_CSS Dir", "Custom_JS Dir": Value Change {
              n99 = event-data() -> ("CtlRef"=w143:refnum<vi>, "NewVal"=w153:i16)  [unwired: 1 in, 1 out]
              n100 = control-ref of="Custom_HTML Dir"() -> (w164:refnum<vi>)
              n101 = control-ref of="Custom_Image Dir"() -> (w163:refnum<vi>)
              n102 = control-ref of="Custom_CSS Dir"() -> (w162:refnum<vi>)
              n103 = control-ref of="Custom_JS Dir"() -> (w161:refnum<vi>)
              n104 = call "VIH Project - Container - Master Rule.vi"() -> ("Rule out"=w151:T16)  [unwired: 11 in]
              n105 = Build Array(w164, w163, w162, w161) -> (w160:refnum<vi>[])
              n106 = Unbundle By Name(w151) -> ("Target Paths.HTML Dir"=w150:path, "Target Paths.Image Dir"=w149:path, "Target Paths.CSS Dir"=w148:path, "Target Paths.JS Dir"=w147:path)
              n107 = Greater Than 0?(x=w153) -> (x > 0?=w142:bool)
              n108 = Search 1D Array(1D array=w160, element=w143) -> (index of element=w145:i32)  [unwired: 1 in]
              n109 = control-ref of="Dst_HTML Dir"() -> (w159:refnum<vi>)
              n110 = control-ref of="Dst_Image Dir"() -> (w158:refnum<vi>)
              n111 = control-ref of="Dst_CSS Dir"() -> (w157:refnum<vi>)
              n112 = control-ref of="Dst_JS Dir"() -> (w156:refnum<vi>)
              n113 = Build Array(w150, w149, w148, w147) -> (w146:path[])
              n114 = Build Array(w159, w158, w157, w156) -> (w155:refnum<vi>[])
              n115 = call "VIH Constant - Default Path Keyword.vi"() -> ("<default> path"=w141:path)  [unwired: 11 in]
              n116 = Index Array(array=w146, index=w145) -> (element=w144:path)
              n117 = Index Array(array=w155, index=w145) -> (element=w154:refnum<vi>)
              n118 = Select(t=w144, s=w142, f=w141) -> (s? t:f=w152:path)
              n119 = disable-structure shown="Disabled" {
                disable-tunnel: w154 -> [w167 _]
                disable-tunnel: w152 -> [w166 _]
                frame Disabled {
                  n120 = property class="Path"(reference=w167, "Value"=w166) -> ()  [unwired: 1 in, 2 out]
                }
                frame Enabled {
                }
              }
            }
            event "VIDescription", "VIDetails": Value Change {
              n121 = event-data() -> ()  [unwired: 1 in, 1 out]
            }
            event Value Change {
              n122 = event-data() -> ()  [unwired: 1 in, 1 out]
            }
            event "CtrlRule List": Value Change {
              n123 = event-data() -> ()  [unwired: 1 in, 1 out]
            }
            event "CtrlRule List": Double Click {
              n124 = event-data() -> ("CtlRef"=w172:refnum<vi>, "Row"=w173:i32)  [unwired: 1 in, 6 out]
              n125 = property class="MCListbox (strict)"(reference=w172) -> ("ItemNames"=w174:string[][])  [unwired: 1 in, 2 out]
              n126 = Index Array(array=w174, index (row)=w173, index (col)=1 ("disabled index (col)")) -> (element=w176:string)
              n127 = Empty String/Path?(string/path=w176) -> (empty?=w177:bool)
              n128 = case shown="False" w177 {
                tunnel: [w180 _] -> w171
                tunnel: w173 -> [w178 _]
                frame False {
                  n129 = Format Into String(format string="CtrlRule: Edit Enum Values = %d;" ("string"), w178) -> (resulting string=w180:string)  [unwired: 2 in, 1 out]
                }
                frame True {
                }
              }
            }
            event "CtrlRule List": Edit Cell {
              n130 = event-data() -> ("String"=w182:string)  [unwired: 1 in, 4 out]
              n131 = local write "CtrlRule_CtrlID"(w182) -> ()
              n132 = Index Array(array=w183) -> (element=w181:i32)  [unwired: 1 in]
              n133 = Format Into String(format string="CtrlRule: Apply = %d;" ("string"), w181) -> (resulting string=w185:string)  [unwired: 2 in, 1 out]
            }
            event "CtrlRule List": Mouse Up {
              n134 = event-data() -> ("CtlRef"=w197:refnum<vi>, "Coords"=w199:T22, "Button"=w198:u16)  [unwired: 1 in, 2 out]
              n135 = property class="MCListbox (strict)"(reference=w197) -> ("ItemSyms"=w187:i32[])  [unwired: 1 in, 2 out]
              n136 = invoke class="MCListbox (strict)" method="Point To Row Column"(reference=w197, "Point"=w199) -> ("CellPosition"=w195:T23, "InGlyph"=w190:bool)  [unwired: 5 in, 5 out]
              n137 = Equal?(x=w198, y=u16 1) -> (x = y?=w191:bool)
              n138 = Array Size(array=w187) -> (size(s)=w194:i32)
              n139 = Unbundle By Name(w195) -> ("Row"=w193:i32)
              n140 = In Range and Coerce(upper limit=w194, x=w193, lower limit=0) -> (coerced(x)=w186:i32, In Range?=w189:bool)
              n141 = Compound Arithmetic op=AND(w190, w191, w189) -> (w188:bool)
              n142 = case shown="True" w188 {
                tunnel: [_ w206] -> w200
                tunnel: w187 -> [_ w213]
                tunnel: w186 -> [_ w203]
                frame False {
                }
                frame True {
                  n143 = Index Array(array=w213, index=w203) -> (element=w211:i32)
                  n144 = Build Array(w203) -> (w202:i32[])
                  n145 = And(x=65535, y=w211) -> (x .and. y?=w210:i32)
                  n146 = Number To Decimal String(number=w202) -> (decimal integer string=w201:string[])  [unwired: 1 in]
                  n147 = Equal?(x=w210, y=37) -> (x = y?=w207:bool)
                  n148 = call "VIH Utility - STR - String from 1D Str Array.vi"("delimiter ('\\n')"="," ("delimiter ('\\n')"), "Array in"=w201) -> ("String out"=w204:string)  [unwired: 5 in]
                  n149 = Format Into String(format string="CtrlRule: Enable = %d ? %s;" ("string"), w207, w204) -> (resulting string=w206:string)  [unwired: 2 in, 1 out]
                }
              }
            }
            event "CtrlRule List": Drag Ended {
              n150 = event-data() -> ("Result"=w214:enum16{"Drop Cancel", "Drop Move", "Drop Copy"})  [unwired: 1 in, 1 out]
              n151 = case shown="\"Drop Move\"" w214 {
                tunnel: [_ "CtrlRule: Dragged;"] -> w215
                frame Default {
                }
                frame "Drop Move" {
                }
              }
            }
            event "CtrlRule List": Shortcut Menu Activation? {
              n152 = event-data() -> ()  [unwired: 1 in, 4 out]
              n153 = event-data("Discard?"=TRUE) -> ()  [unwired: 1 in, 1 out]
            }
            event "%CtrlRule_Add", "%CtrlRule_Remove": Value Change {
              n154 = event-data() -> ()  [unwired: 1 in, 1 out]
              n155 = Build Array("%CtrlRule_Add", "%CtrlRule_Remove") -> (w223:bool[])
              n156 = Search 1D Array(1D array=w223, element=TRUE) -> (index of element=w221:i32)  [unwired: 1 in]
              n157 = Pick Line(multi-line string="CtrlRule: Add;              Key Focus = CtrlRule Control ID;\nCtrlRule: Remove;       Key Focus = CtrlRule List;" ("string"), line index=w221) -> (output string=w219:string)  [unwired: 1 in]
            }
            event "%CtrlRule_Import", "%CtrlRule_Paste", "%CtrlRule_Copy": Value Change {
              n158 = event-data() -> ()  [unwired: 1 in, 1 out]
              n159 = Build Array("%CtrlRule_Import", "%CtrlRule_Paste", "%CtrlRule_Copy") -> (w233:bool[])
              n160 = Search 1D Array(1D array=w233, element=TRUE) -> (index of element=w231:i32)  [unwired: 1 in]
              n161 = Pick Line(multi-line string="CtrlRule: Import = VI;    Key Focus = CtrlRule List;\nCtrlRule: Import = CB;   Key Focus = CtrlRule List;\nCtrlRule: Export = CB;   Key Focus = CtrlRule List;" ("string"), line index=w231) -> (output string=w229:string)  [unwired: 1 in]
            }
            event "CtrlRule_CtrlID", "CtrlRule_CustomRule", "CtrlRule_Description", "CtrlRule_CustomName": Value Change {
              n162 = event-data() -> ()  [unwired: 1 in, 1 out]
              n163 = Index Array(array=w235) -> (element=w237:i32)  [unwired: 1 in]
              n164 = Array Size(array=w235) -> (size(s)=w240:i32)
              n165 = Equal?(x=w240, y=1) -> (x = y?=w238:bool)
              n166 = Select(t=w237, s=w238, f=-1) -> (s? t:f=w234:i32)
              n167 = Format Into String(format string="CtrlRule: Apply = %d;" ("string"), w234) -> (resulting string=w242:string)  [unwired: 2 in, 1 out]
            }
            event "%CtrlRule_Edit_Enum": Value Change {
              n168 = event-data() -> ()  [unwired: 1 in, 1 out]
              n169 = Index Array(array=w245) -> (element=w244:i32)  [unwired: 1 in]
              n170 = Array Size(array=w245) -> (size(s)=w247:i32)
              n171 = Equal?(x=w247, y=1) -> (x = y?=w243:bool)
              n172 = case shown="True" w243 {
                tunnel: [_ w251] -> w248
                tunnel: w244 -> [_ w249]
                frame False {
                }
                frame True {
                  n173 = Format Into String(format string="CtrlRule: Edit Enum Values = %d;" ("string"), w249) -> (resulting string=w251:string)  [unwired: 2 in, 1 out]
                }
              }
            }
            event "CSS List": Value Change {
              n174 = event-data() -> ()  [unwired: 1 in, 1 out]
            }
            event "CSS List": Drag Ended {
              n175 = event-data() -> ("Result"=w253:enum16{"Drop Cancel", "Drop Move", "Drop Copy"})  [unwired: 1 in, 1 out]
              n176 = case shown="\"Drop Move\"" w253 {
                tunnel: [_ "CSS List: Dragged;"] -> w254
                frame Default {
                }
                frame "Drop Move" {
                }
              }
            }
            event "CSS List": Shortcut Menu Activation? {
              n177 = event-data() -> ()  [unwired: 1 in, 4 out]
              n178 = event-data("Discard?"=TRUE) -> ()  [unwired: 1 in, 1 out]
            }
            event "%CSS List_Add", "%CSS List_Remove": Value Change {
              n179 = event-data() -> ()  [unwired: 1 in, 1 out]
              n180 = Build Array("%CSS List_Add", "%CSS List_Remove") -> (w264:bool[])
              n181 = Search 1D Array(1D array=w264, element=TRUE) -> (index of element=w262:i32)  [unwired: 1 in]
              n182 = Pick Line(multi-line string="CSS List: Add;         Key Focus = CSS List;\nCSS List: Remove;  Key Focus = CSS List;", line index=w262) -> (output string=w258:string)  [unwired: 1 in]
            }
            event "JS List": Value Change {
              n183 = event-data() -> ()  [unwired: 1 in, 1 out]
            }
            event "JS List": Drag Ended {
              n184 = event-data() -> ("Result"=w266:enum16{"Drop Cancel", "Drop Move", "Drop Copy"})  [unwired: 1 in, 1 out]
              n185 = case shown="\"Drop Move\"" w266 {
                tunnel: [_ "JS List: Dragged;"] -> w267
                frame Default {
                }
                frame "Drop Move" {
                }
              }
            }
            event "JS List": Shortcut Menu Activation? {
              n186 = event-data() -> ()  [unwired: 1 in, 4 out]
              n187 = event-data("Discard?"=TRUE) -> ()  [unwired: 1 in, 1 out]
            }
            event "%JS List_Add", "%JS List_Remove": Value Change {
              n188 = event-data() -> ()  [unwired: 1 in, 1 out]
              n189 = Build Array("%JS List_Add", "%JS List_Remove") -> (w277:bool[])
              n190 = Search 1D Array(1D array=w277, element=TRUE) -> (index of element=w275:i32)  [unwired: 1 in]
              n191 = Pick Line(multi-line string="JS List: Add;         Key Focus = JS List;\nJS List: Remove;  Key Focus = JS List;", line index=w275) -> (output string=w271:string)  [unwired: 1 in]
            }
            event Value Change {
              n192 = event-data() -> ()  [unwired: 1 in, 1 out]
              n193 = control-ref of="VIDescription"() -> (w279:refnum<vi>)
              n194 = Build Array("%VIDscr_Insert_HREF", "%VIDscr_Insert_<B>", "%VIDscr_Insert_<I>", "%VIDscr_Insert_<U>") -> (w285:T4[])
              n195 = Search 1D Array(1D array=w285, element=TRUE) -> (index of element=w287:i32)  [unwired: 1 in]
              n196 = Increment(x=w287) -> (x+1=w288:i32)
              n197 = Type Cast(type=enum32{"nop", "<a>", "<b>", "<i>", "<u>"}."nop" ("cmd"), x=w288) -> (*(type *) &x=w290:enum32{"nop", "<a>", "<b>", "<i>", "<u>"})
              n198 = call "VIH UI - Insert HTML Tag to String.vi"("cmd"=w290, "Project Tree"=w284, "Str Refnum"=w279) -> ("dup Str Refnum"=w278:refnum<vi>)  [unwired: 8 in]
              n199 = call "VIH UI - Undo Focused Control - Core.vi"("Ctl Refnum"=w278) -> ()  [unwired: 8 in, 3 out]
            }
            event Value Change {
              n200 = event-data() -> ()  [unwired: 1 in, 1 out]
              n201 = control-ref of="VIDetails"() -> (w292:refnum<vi>)
              n202 = Build Array("%VIDetails_Insert_HREF", "%VIDetails_Insert_<B>", "%VIDetails_Insert_<I>", "%VIDetails_Insert_<U>") -> (w298:T4[])
              n203 = Search 1D Array(1D array=w298, element=TRUE) -> (index of element=w300:i32)  [unwired: 1 in]
              n204 = Increment(x=w300) -> (x+1=w301:i32)
              n205 = Type Cast(type=enum32{"nop", "<a>", "<b>", "<i>", "<u>"}."nop" ("cmd"), x=w301) -> (*(type *) &x=w303:enum32{"nop", "<a>", "<b>", "<i>", "<u>"})
              n206 = call "VIH UI - Insert HTML Tag to String.vi"("cmd"=w303, "Project Tree"=w297, "Str Refnum"=w292) -> ("dup Str Refnum"=w291:refnum<vi>)  [unwired: 8 in]
              n207 = call "VIH UI - Undo Focused Control - Core.vi"("Ctl Refnum"=w291) -> ()  [unwired: 8 in, 3 out]
            }
            event Value Change {
              n208 = event-data() -> ()  [unwired: 1 in, 1 out]
              n209 = control-ref of="CtrlRule_Description"() -> (w310:refnum<vi>)
              n210 = Build Array("%CtrlRule_Insert_HREF", "%CtrlRule_Insert_<B>", "%CtrlRule_Insert_<I>", "%CtrlRule_Insert_<U>") -> (w311:T4[])
              n211 = Search 1D Array(1D array=w311, element=TRUE) -> (index of element=w313:i32)  [unwired: 1 in]
              n212 = Increment(x=w313) -> (x+1=w314:i32)
              n213 = Type Cast(type=enum32{"nop", "<a>", "<b>", "<i>", "<u>"}."nop" ("cmd"), x=w314) -> (*(type *) &x=w316:enum32{"nop", "<a>", "<b>", "<i>", "<u>"})
              n214 = call "VIH UI - Insert HTML Tag to String.vi"("cmd"=w316, "Project Tree"=w309, "Str Refnum"=w310) -> ("dup Str Refnum"=w304:refnum<vi>)  [unwired: 8 in]
              n215 = call "VIH UI - Undo Focused Control - Core.vi"("Ctl Refnum"=w304) -> ()  [unwired: 8 in, 3 out]
            }
            event "ProductInfoText": Shortcut Menu Activation? {
              n216 = event-data() -> ("Type"=w321:T24, "CtlRef"=w320:refnum<vi>, "MenuRef"=w319:refnum<k9>)  [unwired: 1 in, 1 out]
              n217 = call "VIH UI - String Shortcut Menu Handler.vi"("Project Tree"=w318, "mode"=enum16{"basic", "format 1", "format 2"}."format 2", "menu"=w319, "Str Refnum"=w320, "Type"=w321) -> ()  [unwired: 7 in]
              n218 = event-data() -> ()  [unwired: 2 in, 1 out]
            }
            event "ProductInfoText": Shortcut Menu Selection (User) {
              n219 = event-data() -> ("Type"=w325:T24, "CtlRef"=w324:refnum<vi>, "ItemTag"=w323:string)  [unwired: 1 in, 1 out]
              n220 = call "VIH UI - String Shortcut Menu Handler.vi"("Project Tree"=w322, "Menu tag"=w323, "Str Refnum"=w324, "Type"=w325) -> ()  [unwired: 8 in]
            }
            event "VIDescription", "VIDetails", "CtrlRule_Description": Shortcut Menu Activation? {
              n221 = event-data() -> ("Type"=w330:T24, "CtlRef"=w329:refnum<vi>, "MenuRef"=w328:refnum<k9>)  [unwired: 1 in, 1 out]
              n222 = call "VIH UI - String Shortcut Menu Handler.vi"("Project Tree"=w327, "mode"=enum16{"basic", "format 1", "format 2"}."format 1", "menu"=w328, "Str Refnum"=w329, "Type"=w330) -> ()  [unwired: 7 in]
              n223 = event-data() -> ()  [unwired: 2 in, 1 out]
            }
            event "VIDescription", "VIDetails", "CtrlRule_Description": Shortcut Menu Selection (User) {
              n224 = event-data() -> ("Type"=w334:T24, "CtlRef"=w333:refnum<vi>, "ItemTag"=w332:string)  [unwired: 1 in, 1 out]
              n225 = call "VIH UI - String Shortcut Menu Handler.vi"("Project Tree"=w331, "Menu tag"=w332, "Str Refnum"=w333, "Type"=w334) -> ()  [unwired: 8 in]
            }
            event "Comments", "CtrlRule_CtrlID", "CtrlRule_CustomName": Shortcut Menu Activation? {
              n226 = event-data() -> ("Type"=w339:T24, "CtlRef"=w338:refnum<vi>, "MenuRef"=w337:refnum<k9>)  [unwired: 1 in, 1 out]
              n227 = call "VIH UI - String Shortcut Menu Handler.vi"("Project Tree"=w336, "mode"=enum16{"basic", "format 1", "format 2"}."basic", "menu"=w337, "Str Refnum"=w338, "Type"=w339) -> ()  [unwired: 7 in]
              n228 = event-data() -> ()  [unwired: 2 in, 1 out]
            }
            event "Comments", "CtrlRule_CtrlID", "CtrlRule_CustomName": Shortcut Menu Selection (User) {
              n229 = event-data() -> ("Type"=w343:T24, "CtlRef"=w342:refnum<vi>, "ItemTag"=w341:string)  [unwired: 1 in, 1 out]
              n230 = call "VIH UI - String Shortcut Menu Handler.vi"("Project Tree"=w340, "Menu tag"=w341, "Str Refnum"=w342, "Type"=w343) -> ()  [unwired: 8 in]
            }
          }
        }
      }
      frame "STARTUP" {
        w354 = i32[] [] ("CSS List")
        w355 = u32 16777216
        w361 = T25 {"Horizontal"=0, "Vertical"=0} ("Origin")
        w357 = T26 {"Left"=2, "Top"=0} ("Position")
        w364 = 1 ("CategoryList")
        n231 = control-ref of="Category List"() -> (w345:refnum<vi>)
        n232 = control-ref of="JS List"() -> (w352:refnum<vi>)
        n233 = control-ref of="CSS List"() -> (w353:refnum<vi>)
        n234 = property on="Pane-Top" class="Pane"("Origin"=w361) -> ()  [unwired: 2 in, 2 out]
        n235 = local write "Category List"(w364) -> ()
        n236 = local write "CSS List"(w354) -> ()
        n237 = property on="Pane-Left" class="Pane"("Origin"=w361) -> ()  [unwired: 2 in, 2 out]
        n238 = Build Array(w353, w352) -> (w351:refnum<vi>[])
        n239 = property on="Pane-Right" class="Pane"("Origin"=w361) -> ("Decos[]"=w360:refnum<vi>[])  [unwired: 2 in, 2 out]
        n240 = local write "JS List"(w354) -> ()
        n241 = local write "Tab Control"(w364) -> ()
        n242 = disable-structure shown="Disabled" {
          disable-tunnel: w351 -> [w369 _ _]
          disable-tunnel: w345 -> [_ w378 _]
          frame Disabled {
            n243 = call "VIH Utility - DEV - Get DevTime Utility VIs Folder.vi"("Utility VI Name"="Utility - Set File List Icons.vi") -> ("error out"=w374:errorcluster, "Utility VIs Path"=w373:path)  [unwired: 8 in, 1 out]
            n244 = Open VI Reference(type specifier VI Refnum (for type only)=refnum<vi> refnum, vi path=w373, error in (no error)=w374) -> (vi reference=w376:refnum<vi>, error out=w377:errorcluster)  [unwired: 3 in]
            n245 = call-by-ref "?"(reference=w376, error in=w377, "MCListbox Refnums"=w369) -> (reference out=w371:refnum<vi>, error out=w372:errorcluster, 0:"error out"=w368:errorcluster)  [unwired: 10 in]
            n246 = Close Reference(reference=w371, error in (no error)=w372) -> (error out=w367:errorcluster)
            n247 = Select(t=w367, s=w367, f=w368) -> (s? t:f=w370:errorcluster)
            n248 = call <vilib>:"Simple Error Handler.vi"("error in (no error)"=w370) -> ()  [unwired: 4 in, 5 out]
          }
          frame Disabled {
            n249 = call "VIH Utility - DEV - Get DevTime Utility VIs Folder.vi"("Utility VI Name"="Utility - Set Category List Text & Icons.vi") -> ("error out"=w386:errorcluster, "Utility VIs Path"=w385:path)  [unwired: 8 in, 1 out]
            n250 = Open VI Reference(type specifier VI Refnum (for type only)=refnum<vi> refnum, vi path=w385, error in (no error)=w386) -> (vi reference=w388:refnum<vi>, error out=w389:errorcluster)  [unwired: 3 in]
            n251 = call-by-ref "?"(reference=w388, error in=w389, "LstBox Refnum"=w378) -> (reference out=w383:refnum<vi>, error out=w384:errorcluster, 0:"error out"=w381:errorcluster)  [unwired: 10 in]
            n252 = Close Reference(reference=w383, error in (no error)=w384) -> (error out=w380:errorcluster)
            n253 = Select(t=w380, s=w380, f=w381) -> (s? t:f=w382:errorcluster)
            n254 = call <vilib>:"Simple Error Handler.vi"("error in (no error)"=w382) -> ()  [unwired: 4 in, 5 out]
          }
          frame Enabled {
          }
        }
        n255 = local write "CtrlRule List"(w354) -> ()
        n256 = Index Array(array=w360) -> (element=w362:refnum<vi>)  [unwired: 1 in]
        n257 = property class="Decor"(reference=w362, "Position"=w357) -> (error out=w358:errorcluster)  [unwired: 1 in, 1 out]
        n258 = property on="Tab Control" class="TabCtl (strict)"(error in=w358, "Position"=w357, "BG Color"=w355, "FG Color"=w355, "Tabs Visible?"=FALSE, "SkipTabbing"=TRUE ("Skip When Tabbing")) -> (error out=w359:errorcluster)  [unwired: 1 in, 1 out]
        n259 = Close Reference(reference=w360, error in (no error)=w359) -> ()  [unwired: 1 out]
        n260 = property class="VI"() -> ("FP.State"=w348:T10)  [unwired: 2 in, 2 out]
        n261 = call "VIH Debug Flag Container.vi"() -> ("Debug Mode"=w349:bool)  [unwired: 11 in]
        n262 = Equal?(x=w348, y=T10."Standard" ("Front Panel Window:State")) -> (x = y?=w346:bool)
        n263 = Or(x=w346, y=w349) -> (x .or. y?=w350:bool)
        n264 = property on="%STOP" class="Bool"("Visible"=w350) -> ()  [unwired: 2 in, 2 out]
        n265 = property on="%UPDATE" class="Bool"("Visible"=w350) -> ()  [unwired: 2 in, 2 out]
      }
      frame "INIT" {
      }
      frame "EXIT" {
        w395 = i32[] [] ("Item Symbols")
        w396 = string[][] [] ("Item Names")
        w397 = T27 {"Row"=0, "Column"=0} ("Top Left Visible Cell")
        n266 = control-ref of="Tab Control"() -> (w394:refnum<vi>)
        n267 = property class="TabCtl (strict)"(reference=w394, "DisabledEnum"=T11."Enabled" ("Disabled")) -> ("Pages"=w393:refnum<vi>[])  [unwired: 1 in, 2 out]
        n268 = property on="CtrlRule List" class="MCListbox (strict)"("TopLeft"=w397, "Value"=w395, "ItemNames"=w396, "ItemSyms"=w395) -> ()  [unwired: 2 in, 2 out]
        n269 = for {
          tunnel: w393 -> [w403] mode=indexing
          n270 = property class="Page"(reference=w403) -> (reference out=w401:refnum<vi>, "Controls on Page[]"=w402:refnum<vi>[])  [unwired: 1 in, 1 out]
          n271 = for {
            tunnel: w402 -> [w407] mode=indexing
            shift-right: [w404] -> w400
            shift-left: w401 -> [w404]
            n272 = property class="Ctl"(reference=w407, "DisabledEnum"=T11."Enabled" ("Disabled")) -> (reference out=w405:refnum<vi>)  [unwired: 1 in, 1 out]
            n273 = Close Reference(reference=w405) -> ()  [unwired: 1 in, 1 out]
          }
          n274 = Close Reference(reference=w400) -> ()  [unwired: 1 in, 1 out]
        }
        n275 = property on="CSS List" class="MCListbox (strict)"("TopLeft"=w397, "Value"=w395, "ItemNames"=w396, "ItemSyms"=w395) -> ()  [unwired: 2 in, 2 out]
        n276 = property on="JS List" class="MCListbox (strict)"("TopLeft"=w397, "Value"=w395, "ItemNames"=w396, "ItemSyms"=w395) -> ()  [unwired: 2 in, 2 out]
      }
      frame "HALT" {
        w408 = TRUE ("Visible")
        w409 = u32 16777238
        n277 = Unregister For Events(event registration refnum=w416) -> (error out=w414:errorcluster)  [unwired: 1 in]
        n278 = Destroy User Event(user event=w415, error in=w414) -> (error out=w412:errorcluster)
        n279 = Release Queue(queue=w413, error in (no error)=w412) -> ()  [unwired: 1 in, 3 out]
        n280 = property on="%STOP" class="Bool"("Visible"=w408) -> ()  [unwired: 2 in, 2 out]
        n281 = property on="Tab Control" class="TabCtl (strict)"("BG Color"=w409, "FG Color"=w409, "Tabs Visible?"=TRUE) -> ()  [unwired: 2 in, 2 out]
        n282 = property on="%UPDATE" class="Bool"("Visible"=w408) -> ()  [unwired: 2 in, 2 out]
      }
      frame "------------------------------ 1" {
      }
      frame "UPDATE" {
        n283 = Unbundle(w441) -> ("Array out"=w430:string[])  [unwired: 1 out]
        n284 = case shown="Default" w431 {
          selector: w431 -> [w458 _]
          tunnel: w430 -> [_ w460]
          tunnel: [w457 w460] -> w428
          frame Default {
            n285 = call "VIH Utility - STR - String to 1D Str Array.vi"("delimiter ('\\n')"="|" ("delimiter ('\\n')"), "String in"=w458) -> ("Array out"=w457:string[])  [unwired: 5 in]
          }
          frame "REFRESH" {
          }
        }
        n286 = control-ref of="ProductInfoText"() -> (w425:refnum<vi>)
        n287 = control-ref of="Comments"() -> (w424:refnum<vi>)
        n288 = control-ref of="Out File Name"() -> (w423:refnum<vi>)
        n289 = control-ref of="VIDescription"() -> (w422:refnum<vi>)
        n290 = control-ref of="VIDetails"() -> (w421:refnum<vi>)
        n291 = Array Size(array=w428) -> (size(s)=w437:i32)
        n292 = Build Array(w425, w424, w423, w422, w421) -> (w426:refnum<vi>[])
        n293 = Index Array(array=w428) -> (element=w440:string)  [unwired: 1 in]
        n294 = Greater?(x=w437, y=1) -> (0:w429:bool)
        n295 = for {
          tunnel: w426 -> [w446] mode=indexing
          n296 = property on="Property Node" class="Str"(reference=w446, "Text.Selection"=T12 {"Selection Start"=0, "Selection End"=0}) -> ()  [unwired: 1 in, 2 out]
        }
        n297 = call "VIH Project Tree - Item Tag - Parse.vi"("Tree Item Tag"=w440) -> ("Item File Path"=w438:path, "Item Type"=w434:T28)  [unwired: 8 in, 1 out]
        n298 = case shown="True" w429 {
          selector: w429 -> [w448 _]
          tunnel: [w448 w450] -> w427
          tunnel: w428 -> [_ w449]
          frame False {
          }
          frame True {
            n299 = for {
              tunnel: [w456] -> w454 mode=indexing
              tunnel: w449 -> [w455] mode=indexing
              n300 = call "VIH Project Tree - Item Tag - Parse.vi"("Tree Item Tag"=w455) -> ("Item File Path"=w456:path)  [unwired: 8 in, 2 out]
            }
            n301 = call "VIH Utility - FILE - Remove Duplicated Paths from 1D Array.vi"("Array in"=w454) -> ("Array out"=w451:path[])  [unwired: 9 in, 1 out]
            n302 = Array Size(array=w451) -> (size(s)=w452:i32)
            n303 = Greater?(x=w452, y=1) -> (0:w450:bool)
          }
        }
        n304 = call "VIH Project - Container - Item Rules.vi"("Item Path"=w438) -> ("Item Rule out"=w439:T29)  [unwired: 6 in, 4 out]
        n305 = case shown="\"Proj Files\"" w434 {
          tunnel: [FALSE TRUE TRUE TRUE TRUE TRUE TRUE TRUE] -> w433
          frame Default {
          }
          frame "<Invalid>" {
          }
          frame "Project" {
          }
          frame "Proj Files" {
          }
          frame "Proj Rules" {
          }
          frame "File Group" {
          }
          frame "Rule Group" {
          }
          frame "LV Func" {
          }
        }
        n306 = Or(x=w427, y=w433) -> (x .or. y?=w432:bool)
        n307 = call "VIH Utility - UI - Boolean to Control Disable Status.vi"("Status in"=w432) -> ("Control Disable if True"=w435:u8)  [unwired: 3 in, 1 out]
        n308 = Bundle("Array out"=w428, "Item Rule out"=w439) -> (w442:T32)  [unwired: 1 in]
        n309 = property on="Tab Control" class="TabCtl (strict)"("DisabledEnum"=w435) -> ()  [unwired: 2 in, 2 out]
        n310 = Concatenate Strings("Update Category;\n\nSet Busy = ON;\n\nUpdate: UI;\nUpdate: Product Info;\nUpdate: General;\nUpdate: Target Paths;\nUpdate: Templates;\nUpdate: CSS List = INIT;\nUpdate: JS List = INIT;\nUpdate: Item Rules;\nUpdate: Control Rules = INIT;\n\nCSS List: Update Controls;\nJS List: Update Controls;\nCtrlRule: Update Controls = INIT;\n\nSet Busy = OFF;" ("string"), w445) -> (w444:string)
      }
      frame "Globals" {
        n311 = case shown="\"SET\"" w470 {
          tunnel: [w475 w481 w487] -> w473
          tunnel: w472 -> [w475 w480 w487]
          tunnel: w469 -> [w474 _ _]
          frame Default {
            n312 = One Button Dialog(message=w474) -> ()  [unwired: 1 in, 1 out]
          }
          frame "GET" {
            n313 = Unbundle(w480) -> ("Array out"=w479:string[])  [unwired: 1 out]
            n314 = Index Array(array=w479) -> (element=w478:string)  [unwired: 1 in]
            n315 = call "VIH Project Tree - Item Tag - Parse.vi"("Tree Item Tag"=w478) -> ("Item File Path"=w476:path)  [unwired: 8 in, 2 out]
            n316 = call "VIH Project - Container - Item Rules.vi"("Item Path"=w476) -> ("Item Rule out"=w477:T29)  [unwired: 6 in, 4 out]
            n317 = Bundle("Array out"=w479, "Item Rule out"=w477) -> (w481:T32)  [unwired: 1 in]
          }
          frame "SET" {
            n318 = Unbundle(w487) -> ("Array out"=w486:string[], "Item Rule out"=w484:T29)
            n319 = Index Array(array=w486) -> (element=w485:string)  [unwired: 1 in]
            n320 = call "VIH Project Tree - Item Tag - Parse.vi"("Tree Item Tag"=w485) -> ("Item File Path"=w483:path)  [unwired: 8 in, 2 out]
            n321 = call "VIH Project - Container - Item Rules.vi"("cmd (get)"=T13."set", "Item Rule"=w484, "Item Path"=w483) -> ()  [unwired: 4 in, 5 out]
          }
        }
      }
      frame "Update Category" {
        n322 = Unbundle(w491) -> ("Array out"=w490:string[])  [unwired: 1 out]
        n323 = property on="Category List" class="LstBox (strict)"() -> ("Item Names"=w495:string[])  [unwired: 2 in, 2 out]
        n324 = Index Array(array=w490) -> (element=w489:string)  [unwired: 1 in]
        n325 = Empty String/Path?(string/path=w489) -> (empty?=w488:bool)
        n326 = Index Array(array=w495, index=w494) -> (element=w493:string)
        n327 = case shown="False" w488 {
          tunnel: w493 -> [w504 w518]
          tunnel: [w503 w518] -> w492
          tunnel: w489 -> [w498 _]
          frame False {
            n328 = call "VIH Project Tree - Item Tag - Parse.vi"("Tree Item Tag"=w498) -> ("Item Type"=w502:T28)  [unwired: 8 in, 2 out]
            n329 = call "VIH Project Tree - Item Type to Palette Item Type.vi"("Tree Item Type"=w502) -> ("PolyVI Instance VI"=w499:bool, "Item/File Type"=w501:T33)  [unwired: 9 in]
            n330 = case shown="\"VI\"" w501 {
              tunnel: ["Invalid File" "File" w510 "Palette" "Built-In Function" "Express VI" "Polymorphic VI" "Control" "HTML File"] -> w500
              tunnel: w499 -> [_ _ w509 _ _ _ _ _ _]
              frame "<Invalid>" {
              }
              frame "<unknown>" {
              }
              frame "VI" {
                (unwired) "Instrument"
                n331 = Select(t="PolyVI Instance VI", s=w509, f="VI") -> (s? t:f=w510:string)
              }
              frame "Menu" {
              }
              frame "LV Func" {
              }
              frame "Express VI" {
              }
              frame "Poly VI" {
              }
              frame "CTL" {
              }
              frame "HTML" {
              }
            }
            n332 = Concatenate Strings(w500, " : ", w504) -> (w503:string)
          }
          frame True {
          }
        }
        "CategoryTitle" <- w492
        n333 = To Unsigned Long Integer(number=w494) -> (unsigned 32bit integer=w496:u32)
        n334 = local write "Tab Control"(w496) -> ()
      }
      frame "Set Busy" {
        n335 = case shown="\"ON\"" w519 {
          frame "OFF", Default {
            n336 = call <vilib>:"Unset Busy.vi"() -> ()  [unwired: 11 in, 1 out]
          }
          frame "ON" {
            n337 = call <vilib>:"Set Busy.vi"() -> ()  [unwired: 10 in, 2 out]
          }
        }
      }
      frame "Key Focus" {
        n338 = case shown="\"Category List\"" w523 {
          selector: w523 -> [w532 _ _ _ _ _]
          tunnel: [w532 _ _ _ _ _] -> w522
          frame Default {
          }
          frame "CtrlRule Control ID" {
            n339 = property on="CtrlRule_CtrlID" class="Str"("Key Focus"=TRUE, "Text.Selection End"=u32 9999 ("Text.Selection:End"), "Text.Selection Start"=u32 0 ("Text.Selection:Start")) -> ()  [unwired: 2 in, 2 out]
          }
          frame "CtrlRule List" {
            n340 = property on="CtrlRule List" class="MCListbox (strict)"("Key Focus"=TRUE) -> ()  [unwired: 2 in, 2 out]
          }
          frame "CSS List" {
            n341 = property on="CSS List" class="MCListbox (strict)"("Key Focus"=TRUE) -> ()  [unwired: 2 in, 2 out]
          }
          frame "JS List" {
            n342 = property on="JS List" class="MCListbox (strict)"("Key Focus"=TRUE) -> ()  [unwired: 2 in, 2 out]
          }
          frame "Category List" {
            n343 = property on="Category List" class="LstBox (strict)"("Key Focus"=TRUE) -> ()  [unwired: 2 in, 2 out]
          }
        }
        n344 = stacked-sequence {
          tunnel: w522 -> [_]
          frame #0 {
            n345 = control-ref of="CSS List"() -> (w528:refnum<vi>)
            n346 = control-ref of="JS List"() -> (w527:refnum<vi>)
            n347 = control-ref of="CtrlRule List"() -> (w526:refnum<vi>)
            n348 = control-ref of="Category List"() -> (w529:refnum<vi>)
            n349 = Build Array(w528, w527, w526) -> (w530:refnum<vi>[])
            n350 = for {
              tunnel: w530 -> [w531] mode=indexing
              n351 = call "VIH Utility - UI - Key Focus & Selection Color (MC Listbox).vi"("MCListbox Refnum"=w531) -> ()  [unwired: 8 in, 3 out]
            }
            n352 = call "VIH Utility - UI - Key Focus & Selection Color (Listbox).vi"("LstBox Refnum"=w529) -> ()  [unwired: 8 in, 3 out]
          }
        }
      }
      frame "------------------------------ 2" {
      }
      frame "Update: UI" {
        n353 = Unbundle(w546) -> ("Array out"=w545:string[])  [unwired: 1 out]
        n354 = Index Array(array=w545) -> (element=w544:string)  [unwired: 1 in]
        n355 = call "VIH Project Tree - Item Tag - Parse.vi"("Tree Item Tag"=w544) -> ("Item File Path"=w543:path)  [unwired: 8 in, 2 out]
        n356 = Strip Path(path=w543) -> (name=→"File Name":string)  [unwired: 1 out]
      }
      frame "Update: Product Info" {
        n357 = Unbundle(w574) -> ("Array out"=w572:string[], "Item Rule out"=w573:T29)
        n358 = Index Array(array=w572) -> (element=w570:string)  [unwired: 1 in]
        n359 = Unbundle By Name(w573) -> ("ProductInfoMode"=w562:T2, "ProductInfoText"=w561:string)
        n360 = call "VIH Project - Container - Product Info.vi"() -> ("Product Info out"=w556:T34)  [unwired: 11 in]
        n361 = call "VIH Project Tree - Item Tag - Parse.vi"("Tree Item Tag"=w570) -> ("Item Type"=w571:T28)  [unwired: 8 in, 2 out]
        n362 = Unbundle By Name(w556) -> ("ProductName"=→"PI_Product":string, "Version"=→"PI_Version":string, "Author"=→"PI_Author":string, "Company"=→"PI_Company":string, "Copyright"=→"PI_Copyright":string, "Website"=→"PI_Website":string, "Email"=→"PI_Email":string, "AddInfo"=→"PI_AddInfo":string)
        n363 = call "VIH Project Tree - Item Type to Palette Item Type.vi"("Tree Item Type"=w571) -> ("PolyVI Instance VI"=w568:bool, "Item/File Type"=w569:T33)  [unwired: 9 in]
        n364 = case shown="\"VI\"" w569 {
          tunnel: w568 -> [_ _ w578 _ _ _ _ _ _]
          tunnel: [_ _ w577 TRUE _ _ TRUE _ _] -> w564
          tunnel: [_ _ w576 w580 _ _ w583 _ _] -> w563
          tunnel: w562 -> [_ _ w576 w580 _ _ w583 _ _]
          tunnel: [_ _ w575 w579 _ _ w582 _ _] -> w560
          tunnel: w561 -> [_ _ w575 w579 _ _ w582 _ _]
          frame "<Invalid>" {
          }
          frame "<unknown>" {
          }
          frame "VI" {
            n365 = Not(x=w578) -> (.not. x?=w577:bool)
          }
          frame "Menu" {
          }
          frame "LV Func" {
          }
          frame "Express VI" {
          }
          frame "Poly VI" {
          }
          frame "CTL" {
          }
          frame "HTML" {
          }
        }
        n366 = call "VIH Utility - UI - Boolean to Control Disable Status.vi"("Status in"=w564) -> ("Control Disable if False"=w565:u8)  [unwired: 3 in, 1 out]
        n367 = Not Equal?(x=w563, y=VIH_HelpGen_Typedef_-_Enum_-_Default,Enable,Disable."Enable") -> (x != y?=w567:bool)
        n368 = call "VIH Utility - UI - Boolean to Control Disable Status.vi"("Status in"=w567) -> ("Control Disable if True"=w566:u8)  [unwired: 3 in, 1 out]
        n369 = Max & Min(x=w565, y=w566) -> (max(x,y)=w559:u8)  [unwired: 1 out]
        n370 = property on="ProductInfoMode" class="Ring (strict)"("DisabledEnum"=w565, "Value"=w563) -> ()  [unwired: 2 in, 2 out]
        n371 = property on="ProductInfoText" class="Str"("DisabledEnum"=w559, "Value"=w560) -> ()  [unwired: 2 in, 2 out]
      }
      frame "Update: General" {
        n372 = Unbundle(w619) -> ("Array out"=w612:string[], "Item Rule out"=w618:T29)
        n373 = Unbundle By Name(w618) -> ("OutName"=w616:string, "BuildHelp"=w594:T2, "%Comments"=w595:string, "Flags"=w617:T21)
        n374 = Index Array(array=w612) -> (element=w613:string)  [unwired: 1 in]
        n375 = Unbundle By Name(w617) -> ("Override CSS Files"=w605:bool, "Override JS Files"=w603:bool, "Override Ctl Rules"=w601:bool)
        n376 = Empty String/Path?(string/path=w616) -> (empty?=w607:bool)
        n377 = call "VIH Project Tree - Item Tag - Parse.vi"("Tree Item Tag"=w613) -> ("Item File Path"=w614:path, "Item Type"=w615:T28)  [unwired: 8 in, 1 out]
        n378 = local write "Comments"(w595) -> ()
        n379 = call "VIH Project Tree - Item Type to Palette Item Type.vi"("Tree Item Type"=w615) -> ("PolyVI Instance VI"=w588:bool, "Item/File Type"=w606:T33)  [unwired: 9 in]
        n380 = case shown="\"<unknown>\"" w606 {
          tunnel: [_ _ w627 w631 _ _ w635 _ w638] -> w604
          tunnel: w605 -> [_ _ w627 w631 _ _ w635 _ w638]
          tunnel: [_ _ w626 w630 _ _ w634 _ w639] -> w602
          tunnel: w603 -> [_ _ w626 w630 _ _ w634 _ w639]
          tunnel: [_ _ w625 _ _ _ _ _ _] -> w600
          tunnel: w601 -> [_ _ w625 _ _ _ _ _ _]
          tunnel: [_ _ TRUE _ _ _ _ _ _] -> w599
          tunnel: [_ _ w622 TRUE _ _ TRUE _ TRUE] -> w598
          tunnel: [_ TRUE w622 TRUE _ _ TRUE _ TRUE] -> w593
          tunnel: w588 -> [_ _ w623 _ _ _ _ _ _]
          frame "<Invalid>" {
          }
          frame "<unknown>" {
          }
          frame "VI" {
            (unwired) TRUE
            (unwired) TRUE
            n381 = Not(x=w623) -> (.not. x?=w622:bool)
          }
          frame "Menu" {
          }
          frame "LV Func" {
          }
          frame "Express VI" {
          }
          frame "Poly VI" {
          }
          frame "CTL" {
          }
          frame "HTML" {
          }
        }
        n382 = call "VIH HelpGen - Get Target HTML Filename.vi"("Item File Path"=w614, "Item Type"=w606, "HTML Filename in"=w616) -> ("same as source name"=w611:bool, "HTML Fileame out"=w586:string)  [unwired: 7 in]
        n383 = Select(t="", s=w588, f=w586) -> (s? t:f=w585:string)
        n384 = call "VIH Utility - UI - Boolean to Control Disable Status.vi"("Status in"=w611) -> ("Control Disable if True"=w592:u8)  [unwired: 3 in, 1 out]
        n385 = call "VIH Utility - UI - Boolean to Control Disable Status.vi"("Status in"=w607) -> ("Control Disable if True"=w590:u8)  [unwired: 3 in, 1 out]
        n386 = call "VIH Utility - UI - Boolean to Control Disable Status.vi"("Status in"=w593) -> ("Control Disable if False"=w591:u8)  [unwired: 3 in, 1 out]
        n387 = call "VIH Utility - UI - Boolean to Control Disable Status.vi"("Status in"=w598) -> ("Control Disable if False"=w597:u8)  [unwired: 3 in, 1 out]
        n388 = call "VIH Utility - UI - Boolean to Control Disable Status.vi"("Status in"=w599) -> ("Control Disable if False"=w596:u8)  [unwired: 3 in, 1 out]
        n389 = Not(x=w607) -> (.not. x?=w608:bool)
        n390 = Boolean To (0,1)(Boolean=w608) -> (0, 1=w609:i16)
        n391 = Max & Min(x=w592, y=w591) -> (max(x,y)=w589:u8)  [unwired: 1 out]
        n392 = property on="Custom_OutFile" class="Ring (strict)"("Value"=w609, "DisabledEnum"=w589) -> ()  [unwired: 2 in, 2 out]
        n393 = property on="BuildHelp" class="Enum (strict)"("Value"=w594, "DisabledEnum"=w591) -> ()  [unwired: 2 in, 2 out]
        n394 = property on="Override_CSS Files" class="Bool (strict)"("Value"=w604, "DisabledEnum"=w597) -> ()  [unwired: 2 in, 2 out]
        n395 = property on="Override_JS Files" class="Bool (strict)"("Value"=w602, "DisabledEnum"=w597) -> ()  [unwired: 2 in, 2 out]
        n396 = property on="Override_Ctl Rules" class="Bool (strict)"("Value"=w600, "DisabledEnum"=w596) -> ()  [unwired: 2 in, 2 out]
        n397 = Max & Min(x=w590, y=w589) -> (max(x,y)=w610:u8)  [unwired: 1 out]
        n398 = property on="Out File Name" class="Str"("Value"=w585, "DisabledEnum"=w610) -> ()  [unwired: 2 in, 2 out]
        n399 = property on="CSS List" class="MCListbox (strict)"("DisabledEnum"=w597) -> ()  [unwired: 2 in, 2 out]
        n400 = property on="JS List" class="MCListbox (strict)"("DisabledEnum"=w597) -> ()  [unwired: 2 in, 2 out]
        n401 = property on="CtrlRule List" class="MCListbox (strict)"("DisabledEnum"=w596) -> ()  [unwired: 2 in, 2 out]
      }
      frame "Update: Target Paths" {
        w659 = FALSE ("Allow Empty Path (T)")
        w660 = TRUE ("Ena Empty Path")
        n402 = Unbundle(w692) -> ("Array out"=w669:string[], "Item Rule out"=w691:T29)
        n403 = property on="Out File Name" class="Str"() -> ("Value"=w641:string)  [unwired: 2 in, 2 out]
        n404 = Index Array(array=w669) -> (element=w657:string)  [unwired: 1 in]
        n405 = Unbundle By Name(w691) -> ("Target Paths"=w690:T31)
        n406 = call "VIH Project Tree - Item Tag - Parse.vi"("Tree Item Tag"=w657) -> ("Item File Path"=w640:path, "Item Type"=w650:T28)  [unwired: 8 in, 1 out]
        n407 = call "VIH Project - Get Effective File Rule.vi"("Don't Build Abs Paths (F)"=TRUE, "Ignore Control Rules (F)"=TRUE, "File Path"=w640, "Project Tree"=w656) -> ("Build Root Dir"=w642:path, "Effective File Rule"=w643:T29)  [unwired: 4 in, 2 out]
        "Build Root Dir" <- w642
        n408 = Unbundle By Name(w690) -> ("HTML Dir"=w689:path, "Image Dir"=w682:path, "CSS Dir"=w683:path, "JS Dir"=w684:path)
        n409 = call "VIH Project - Get Effective File Rule - Abs Paths.vi"("Build Root Dir"=w642, "File Rule in"=w643) -> ("File Rule out"=w644:T29)  [unwired: 9 in]
        n410 = call "VIH Project Tree - Item Type to Palette Item Type.vi"("Tree Item Type"=w650) -> ("PolyVI Instance VI"=w649:bool, "Item/File Type"=w647:T33)  [unwired: 9 in]
        n411 = Unbundle By Name(w643) -> ("Target Paths.HTML Dir"=w679:path, "Target Paths.Image Dir"=w672:path, "Target Paths.CSS Dir"=w671:path, "Target Paths.JS Dir"=w670:path)
        n412 = call "VIH Utility - UI - Boolean to Control Disable Status.vi"("Status in"=w649) -> ("Control Disable if True"=w648:u8)  [unwired: 3 in, 1 out]
        n413 = call "VIH UI - Path Indication (with Default).vi"("Ena Empty Path"=w660, "Path"=w683) -> ("Custom"=w675:bool, "Disable"=w686:u8, "Path out"=w676:path)  [unwired: 7 in]
        n414 = call "VIH UI - Path Indication (with Default).vi"("Ena Empty Path"=w660, "Path"=w684) -> ("Custom"=w673:bool, "Disable"=w685:u8, "Path out"=w674:path)  [unwired: 7 in]
        n415 = call "VIH UI - Path Indication (with Default).vi"("Ena Empty Path"=w660, "Path"=w682) -> ("Custom"=w677:bool, "Disable"=w687:u8, "Path out"=w678:path)  [unwired: 7 in]
        n416 = call "VIH UI - Path Indication (with Default).vi"("Ena Empty Path"=w660, "Path"=w689) -> ("Custom"=w680:bool, "Disable"=w688:u8, "Path out"=w681:path)  [unwired: 7 in]
        n417 = Empty String/Path?(string/path=w641) -> (empty?=w645:bool)
        n418 = case shown="False" w645 {
          tunnel: w647 -> [w700 _]
          tunnel: [w698 _] -> w646
          tunnel: w641 -> [w697 _]
          tunnel: w644 -> [w696 _]
          tunnel: w640 -> [w694 _]
          frame False {
            n419 = Unbundle By Name(w696) -> ("Target Paths"=w695:T31)
            n420 = call "VIH HelpGen - Get Target Folder for an Output File.vi"("Item/File Type"=w700, "File Path"=w694, "Target Paths"=w695) -> ("Target Folder"=w699:path)  [unwired: 8 in]
            n421 = Build Path(base path=w699, name or relative path=w697) -> (appended path=w698:path)
          }
          frame True {
          }
        }
        "Out File Path" <- w646
        n422 = Boolean To (0,1)(Boolean=w673) -> (0, 1=w651:i16)
        n423 = Boolean To (0,1)(Boolean=w677) -> (0, 1=w653:i16)
        n424 = Select(t=w681, s=w680, f=w679) -> (s? t:f=w661:path)
        n425 = Boolean To (0,1)(Boolean=w675) -> (0, 1=w652:i16)
        n426 = Select(t=w674, s=w673, f=w670) -> (s? t:f=w664:path)
        n427 = Boolean To (0,1)(Boolean=w680) -> (0, 1=w654:i16)
        n428 = Select(t=w678, s=w677, f=w672) -> (s? t:f=w662:path)
        n429 = Select(t=w676, s=w675, f=w671) -> (s? t:f=w663:path)
        n430 = call "VIH HelpGen - FILE - Build Absolute Path.vi"("Root Path"=w642, "Allow Empty Path (T)"=w659, "Path in"=w661) -> ("Path out"=w665:path)  [unwired: 8 in]
        n431 = call "VIH HelpGen - FILE - Build Absolute Path.vi"("Root Path"=w642, "Allow Empty Path (T)"=w659, "Path in"=w662) -> ("Path out"=w666:path)  [unwired: 8 in]
        n432 = call "VIH HelpGen - FILE - Build Absolute Path.vi"("Root Path"=w642, "Allow Empty Path (T)"=w659, "Path in"=w663) -> ("Path out"=w667:path)  [unwired: 8 in]
        n433 = call "VIH HelpGen - FILE - Build Absolute Path.vi"("Root Path"=w642, "Allow Empty Path (T)"=w659, "Path in"=w664) -> ("Path out"=w668:path)  [unwired: 8 in]
        n434 = property on="Dst_HTML Dir" class="Path"("Value"=w661, "DisabledEnum"=w688, "StartPath"=w665) -> ()  [unwired: 2 in, 2 out]
        n435 = property on="Dst_Image Dir" class="Path"("Value"=w662, "DisabledEnum"=w687, "StartPath"=w666) -> ()  [unwired: 2 in, 2 out]
        n436 = property on="Dst_CSS Dir" class="Path"("Value"=w663, "DisabledEnum"=w686, "StartPath"=w667) -> ()  [unwired: 2 in, 2 out]
        n437 = property on="Dst_JS Dir" class="Path"("Value"=w664, "DisabledEnum"=w685, "StartPath"=w668) -> ()  [unwired: 2 in, 2 out]
        n438 = property on="Custom_HTML Dir" class="Ring (strict)"("Value"=w654, "DisabledEnum"=w648) -> ()  [unwired: 2 in, 2 out]
        n439 = property on="Custom_CSS Dir" class="Ring (strict)"("Value"=w652, "DisabledEnum"=w648) -> ()  [unwired: 2 in, 2 out]
        n440 = property on="Custom_Image Dir" class="Ring (strict)"("Value"=w653, "DisabledEnum"=w648) -> ()  [unwired: 2 in, 2 out]
        n441 = property on="Custom_JS Dir" class="Ring (strict)"("Value"=w651, "DisabledEnum"=w648) -> ()  [unwired: 2 in, 2 out]
      }
      frame "Update: Templates" {
        (unwired) VIH_HelpGen_Typedef_-_Palette_-_Item_Type_Enum."<Invalid>" ("Item/File Type")
        n442 = Unbundle(w715) -> ("Array out"=w710:string[], "Item Rule out"=w714:T29)
        n443 = Unbundle By Name(w714) -> ("Source Paths.Html Template"=w706:path)
        n444 = Index Array(array=w710) -> (element=w709:string)  [unwired: 1 in]
        n445 = call "VIH Project Tree - Item Tag - Parse.vi"("Tree Item Tag"=w709) -> ("Item File Path"=w708:path, "Item Type"=w705:T28)  [unwired: 8 in, 1 out]
        n446 = call "VIH Project Tree - Item Type to Palette Item Type.vi"("Tree Item Type"=w705) -> ("PolyVI Instance VI"=w701:bool, "Item/File Type"=w703:T33)  [unwired: 9 in]
        n447 = case shown="\"VI\", \"Menu\", \"Poly VI\"" w703 {
          tunnel: [_ w728] -> w713
          tunnel: [u32 0 w727] -> w712
          tunnel: [w719 w726] -> w711
          tunnel: w708 -> [_ w725]
          tunnel: w707 -> [_ w724]
          tunnel: w706 -> [_ w723]
          tunnel: [i16 0 w722] -> w704
          tunnel: [w719 w721] -> w702
          tunnel: w701 -> [_ w720]
          frame "<Invalid>", "<unknown>", "LV Func", "Express VI", "CTL", "HTML" {
            w719 = u8 2 ("Disable")
          }
          frame "VI", "Menu", "Poly VI" {
            n448 = case shown="False" w720 {
              tunnel: [w743 _] -> w728
              tunnel: [w742 u32 0] -> w727
              tunnel: [w740 w750] -> w726
              tunnel: w725 -> [w734 _]
              tunnel: w724 -> [w733 _]
              tunnel: w723 -> [w731 _]
              tunnel: [w730 i16 0] -> w722
              tunnel: [u8 0 ("Disable") w750] -> w721
              frame False {
                n449 = call "VIH Project - Get Effective File Rule.vi"("Ignore Control Rules (F)"=TRUE, "File Path"=w734, "Project Tree"=w733) -> ("Effective File Rule"=w732:T29)  [unwired: 5 in, 3 out]
                n450 = Unbundle By Name(w732) -> ("Source Paths.Html Template"=w736:path)
                n451 = call "VIH UI - Path Indication (with Default).vi"("Ena Empty Path"=FALSE, "Path"=w731) -> ("Custom"=w738:bool, "Disable"=w739:u8, "Path out"=w741:path)  [unwired: 7 in]
                n452 = case shown="True" w738 {
                  tunnel: [w744 w748] -> w743
                  tunnel: [_ w747] -> w742
                  tunnel: w741 -> [_ w746]
                  tunnel: [w745 _] -> w740
                  tunnel: w739 -> [w745 _]
                  tunnel: w736 -> [w744 _]
                  frame False {
                  }
                  frame True {
                    n453 = call "VIH UI - Test Path.vi"("Path"=w746) -> ("Color"=w747:u32, "dup Path"=w748:path)  [unwired: 7 in, 2 out]
                  }
                }
                n454 = Boolean To (0,1)(Boolean=w738) -> (0, 1=w730:i16)
              }
              frame True {
                w750 = u8 2 ("Disable")
              }
            }
          }
        }
        n455 = property on="Src_Template" class="Path"("Value"=w713, "Text.TextColor"=w712, "DisabledEnum"=w711) -> ()  [unwired: 2 in, 2 out]
        n456 = property on="Custom_Template" class="Ring (strict)"("Value"=w704, "DisabledEnum"=w702) -> ()  [unwired: 2 in, 2 out]
      }
      frame "Update: CSS List" {
        n457 = Unbundle(w771) -> ("Item Rule out"=w770:T29)  [unwired: 1 out]
        n458 = Unbundle By Name(w770) -> ("Source Paths"=w769:T30)
        n459 = property on="CSS List" class="MCListbox (strict)"() -> ("DisabledEnum"=w757:T11)  [unwired: 2 in, 2 out]
        n460 = Equal To 0?(x=w757) -> (x = 0?=w756:bool)
        n461 = case shown="True" w756 {
          tunnel: w769 -> [_ w774]
          tunnel: [_ w773] -> w760
          frame False {
          }
          frame True {
            n462 = Unbundle By Name(w774) -> ("CSS Files"=w773:path[])
          }
        }
        n463 = Array Size(array=w760) -> (size(s)=w759:i32)
        n464 = for {
          tunnel: w760 -> [w780] mode=indexing
          tunnel: [w779] -> w753 mode=indexing
          tunnel: [w781] -> w768 mode=indexing
          n465 = Path To String(path=w780) -> (string=w782:string)
          n466 = call "VIH UI - Test Path.vi"("Path"=w780) -> ("Symbol"=w779:i32)  [unwired: 7 in, 3 out]
          n467 = Build Array(w782) -> (w781:string[])
        }
        n468 = Not Equal?(x=w753, y=0) -> (x != y?=w755:bool[])
        n469 = call "VIH Utility - UI - Drag and Drop Supporter (w Symbol Indices).vi"("Cmd"=enum16{"make symbols", "test D'n'D"}."make symbols", "Item Symbols"=w753) -> ("Item Symbols out"=w766:i32[])  [unwired: 7 in, 2 out]
        n470 = Or Array Elements(Boolean array=w755) -> (logical OR=w752:bool)
        n471 = control-ref of="CSS List"() -> (w765:refnum<vi>)
        n472 = property on="CSS List" class="MCListbox (strict)"("ItemNames"=w768, "ItemSyms"=w766, "Symbols Vis"=w752) -> (error out=w758:errorcluster)  [unwired: 2 in, 1 out]
        n473 = case shown="\"INIT\"" w761 {
          tunnel: w759 -> [_ w778]
          tunnel: w763 -> [w775 w777]
          tunnel: [w775 w776] -> w762
          tunnel: w758 -> [_ _]
          frame Default {
          }
          frame "INIT" {
            n474 = call "VIH UI - Coerce List Value.vi"("# elements"=w778, "Indices in"=w777) -> ("Indices out"=w776:i32[])  [unwired: 9 in]
            n475 = property on="CSS List" class="MCListbox (strict)"("Value"=w776) -> ()  [unwired: 2 in, 2 out]
          }
        }
        n476 = Index Array(array=w762) -> (element=w764:i32)  [unwired: 1 in]
        n477 = call "VIH Utility - UI - Make Row Visible (MC Listbox).vi"("Row"=w764, "MC Listbox Refnum"=w765) -> ()  [unwired: 8 in, 2 out]
      }
      frame "Update: JS List" {
        n478 = Unbundle(w802) -> ("Item Rule out"=w801:T29)  [unwired: 1 out]
        n479 = Unbundle By Name(w801) -> ("Source Paths"=w800:T30)
        n480 = property on="JS List" class="MCListbox (strict)"() -> ("DisabledEnum"=w788:T11)  [unwired: 2 in, 2 out]
        n481 = Equal To 0?(x=w788) -> (x = 0?=w787:bool)
        n482 = case shown="True" w787 {
          tunnel: w800 -> [_ w805]
          tunnel: [_ w804] -> w792
          frame False {
          }
          frame True {
            n483 = Unbundle By Name(w805) -> ("JS Files"=w804:path[])
          }
        }
        n484 = Array Size(array=w792) -> (size(s)=w791:i32)
        n485 = for {
          tunnel: w792 -> [w811] mode=indexing
          tunnel: [w810] -> w784 mode=indexing
          tunnel: [w812] -> w799 mode=indexing
          n486 = Path To String(path=w811) -> (string=w813:string)
          n487 = call "VIH UI - Test Path.vi"("Path"=w811) -> ("Symbol"=w810:i32)  [unwired: 7 in, 3 out]
          n488 = Build Array(w813) -> (w812:string[])
        }
        n489 = Not Equal?(x=w784, y=0) -> (x != y?=w786:bool[])
        n490 = Or Array Elements(Boolean array=w786) -> (logical OR=w783:bool)
        n491 = call "VIH Utility - UI - Drag and Drop Supporter (w Symbol Indices).vi"("Cmd"=enum16{"make symbols", "test D'n'D"}."make symbols", "Item Symbols"=w784) -> ("Item Symbols out"=w797:i32[])  [unwired: 7 in, 2 out]
        n492 = control-ref of="JS List"() -> (w795:refnum<vi>)
        n493 = property on="JS List" class="MCListbox (strict)"("ItemNames"=w799, "ItemSyms"=w797, "Symbols Vis"=w783) -> (error out=w789:errorcluster)  [unwired: 2 in, 1 out]
        n494 = case shown="\"INIT\"" w794 {
          tunnel: w791 -> [_ w809]
          tunnel: w793 -> [w806 w808]
          tunnel: [w806 w807] -> w790
          tunnel: w789 -> [_ _]
          frame Default {
          }
          frame "INIT" {
            n495 = call "VIH UI - Coerce List Value.vi"("# elements"=w809, "Indices in"=w808) -> ("Indices out"=w807:i32[])  [unwired: 9 in]
            n496 = property on="JS List" class="MCListbox (strict)"("Value"=w807) -> ()  [unwired: 2 in, 2 out]
          }
        }
        n497 = Index Array(array=w790) -> (element=w796:i32)  [unwired: 1 in]
        n498 = call "VIH Utility - UI - Make Row Visible (MC Listbox).vi"("Row"=w796, "MC Listbox Refnum"=w795) -> ()  [unwired: 8 in, 2 out]
      }
      frame "Update: Item Rules" {
        n499 = Unbundle(w842) -> ("Array out"=w840:string[], "Item Rule out"=w841:T29)
        n500 = Index Array(array=w840) -> (element=w838:string)  [unwired: 1 in]
        n501 = Unbundle By Name(w841) -> ("DscrMode"=w836:T7, "Description"=w835:string, "DetailsMode"=w822:T7, "DetailsText"=w821:string)
        n502 = call "VIH Project Tree - Item Tag - Parse.vi"("Tree Item Tag"=w838) -> ("Item Type"=w839:T28)  [unwired: 8 in, 2 out]
        n503 = call "VIH Project Tree - Item Type to Palette Item Type.vi"("Tree Item Type"=w839) -> ("PolyVI Instance VI"=w826:bool, "Item/File Type"=w837:T33)  [unwired: 9 in]
        n504 = case shown="\"Poly VI\"" w837 {
          tunnel: [_ _ w850 w853 _ _ w858 _ _] -> w833
          tunnel: w836 -> [_ _ w850 w853 _ _ w858 _ _]
          tunnel: w835 -> [_ _ w849 w852 _ _ w859 _ _]
          tunnel: [_ _ w849 w852 _ _ w859 _ _] -> w834
          tunnel: [_ _ TRUE TRUE _ _ TRUE _ _] -> w827
          tunnel: w826 -> [_ _ w848 _ _ _ _ _ _]
          tunnel: w822 -> [_ _ w846 _ _ _ w856 _ _]
          tunnel: [_ _ w846 _ _ _ w856 _ _] -> w819
          tunnel: w821 -> [_ _ w845 _ _ _ w855 _ _]
          tunnel: [_ _ w845 _ _ _ w855 _ _] -> w820
          tunnel: [_ _ w844 _ _ _ TRUE _ _] -> w816
          frame "<Invalid>" {
          }
          frame "<unknown>" {
          }
          frame "VI" {
            n505 = Not(x=w848) -> (.not. x?=w844:bool)
          }
          frame "Menu" {
          }
          frame "LV Func" {
          }
          frame "Express VI" {
          }
          frame "Poly VI" {
          }
          frame "CTL" {
          }
          frame "HTML" {
          }
        }
        n506 = call "VIH Utility - UI - Boolean to Control Disable Status.vi"("Status in"=w827) -> ("Control Disable if False"=w828:u8)  [unwired: 3 in, 1 out]
        n507 = call "VIH Utility - UI - Boolean to Control Disable Status.vi"("Status in"=w816) -> ("Control Disable if False"=w817:u8)  [unwired: 3 in, 1 out]
        n508 = Not Equal?(x=w819, y=VIH_HelpGen_Typedef_-_Enum_-_Description_Mode."Custom") -> (x != y?=w824:bool)
        n509 = Not Equal?(x=w833, y=VIH_HelpGen_Typedef_-_Enum_-_Description_Mode."Custom") -> (x != y?=w831:bool)
        n510 = call "VIH Utility - UI - Boolean to Control Disable Status.vi"("Status in"=w824) -> ("Control Disable if True"=w825:u8)  [unwired: 3 in, 1 out]
        n511 = call "VIH Utility - UI - Boolean to Control Disable Status.vi"("Status in"=w831) -> ("Control Disable if True"=w830:u8)  [unwired: 3 in, 1 out]
        n512 = Max & Min(x=w817, y=w825) -> (max(x,y)=w818:u8)  [unwired: 1 out]
        n513 = Max & Min(x=w828, y=w830) -> (max(x,y)=w829:u8)  [unwired: 1 out]
        n514 = property on="VIDscrMode" class="Enum (strict)"("DisabledEnum"=w828, "Value"=w833) -> ()  [unwired: 2 in, 2 out]
        n515 = property on="VIDescription" class="Str"("DisabledEnum"=w829, "Value"=w834) -> ()  [unwired: 2 in, 2 out]
        n516 = property on="VIDetailsMode" class="Enum (strict)"("DisabledEnum"=w817, "Value"=w819) -> ()  [unwired: 2 in, 2 out]
        n517 = property on="VIDetails" class="Str"("DisabledEnum"=w818, "Value"=w820) -> ()  [unwired: 2 in, 2 out]
        n518 = Concatenate Strings("Update: Item Rules 2;", w843) -> (w815:string)
      }
      frame "Update: Item Rules 2" {
        n519 = Unbundle(w877) -> ("Array out"=w875:string[], "Item Rule out"=w876:T29)
        n520 = Index Array(array=w875) -> (element=w873:string)  [unwired: 1 in]
        n521 = Unbundle By Name(w876) -> ("Ctl_DscrMode"=w871:T7, "Ctl_ClustMembers"=w870:T2, "Ctl_EnumValues"=w869:T2, "MenuItemIcons"=w861:T2)
        n522 = call "VIH Project Tree - Item Tag - Parse.vi"("Tree Item Tag"=w873) -> ("Item Type"=w874:T28)  [unwired: 8 in, 2 out]
        n523 = call "VIH Project Tree - Item Type to Palette Item Type.vi"("Tree Item Type"=w874) -> ("Item/File Type"=w872:T33)  [unwired: 9 in, 1 out]
        n524 = case shown="\"<Invalid>\"" w872 {
          tunnel: w871 -> [_ _ w882 _ _ _ _ _ _]
          tunnel: w870 -> [_ _ w881 _ _ _ _ _ _]
          tunnel: w869 -> [_ _ w880 _ _ _ _ _ _]
          tunnel: [_ _ w882 _ _ _ _ _ _] -> w868
          tunnel: [_ _ w881 _ _ _ _ _ _] -> w867
          tunnel: [_ _ w880 _ _ _ _ _ _] -> w866
          tunnel: [_ _ TRUE _ _ _ _ _ _] -> w865
          tunnel: [_ _ _ TRUE _ _ _ _ _] -> w862
          tunnel: w861 -> [_ _ _ w883 _ _ _ _ _]
          tunnel: [_ _ _ w883 _ _ _ _ _] -> w860
          frame "<Invalid>" {
          }
          frame "<unknown>" {
          }
          frame "VI" {
          }
          frame "Menu" {
          }
          frame "LV Func" {
          }
          frame "Express VI" {
          }
          frame "Poly VI" {
          }
          frame "CTL" {
          }
          frame "HTML" {
          }
        }
        n525 = call "VIH Utility - UI - Boolean to Control Disable Status.vi"("Status in"=w865) -> ("Control Disable if False"=w864:u8)  [unwired: 3 in, 1 out]
        n526 = call "VIH Utility - UI - Boolean to Control Disable Status.vi"("Status in"=w862) -> ("Control Disable if False"=w863:u8)  [unwired: 3 in, 1 out]
        n527 = property on="MenuItemIcons" class="Enum (strict)"("DisabledEnum"=w863, "Value"=w860) -> ()  [unwired: 2 in, 2 out]
        n528 = property on="Ctl_DscrMode" class="Enum (strict)"("DisabledEnum"=w864, "Value"=w868) -> ()  [unwired: 2 in, 2 out]
        n529 = property on="Ctl_ClustMembers" class="Enum (strict)"("DisabledEnum"=w864, "Value"=w867) -> ()  [unwired: 2 in, 2 out]
        n530 = property on="Ctl_EnumValues" class="Enum (strict)"("DisabledEnum"=w864, "Value"=w866) -> ()  [unwired: 2 in, 2 out]
      }
      frame "Update: Control Rules" {
        n531 = Unbundle(w900) -> ("Item Rule out"=w899:T29)  [unwired: 1 out]
        n532 = property on="CtrlRule List" class="MCListbox (strict)"() -> ("DisabledEnum"=w886:T11)  [unwired: 2 in, 2 out]
        n533 = Equal To 0?(x=w886) -> (x = 0?=w885:bool)
        n534 = case shown="True" w885 {
          tunnel: w899 -> [_ w903]
          tunnel: [_ w902] -> w892
          frame False {
          }
          frame True {
            n535 = Unbundle By Name(w903) -> ("Control Rules"=w902:T19[])
          }
        }
        n536 = Array Size(array=w892) -> (size(s)=w891:i32)
        n537 = for {
          tunnel: w892 -> [w919] mode=indexing
          tunnel: [w917] -> w898 mode=indexing
          tunnel: [w913] -> w897 mode=indexing
          n538 = Unbundle By Name(w919) -> ("CtrlID"=w918:string, "CustomRule"=w916:bool, "EnumValDscr"=w909:T20[])
          n539 = Empty Array?(array=w909) -> (empty?=w912:bool)
          n540 = Select(t="", s=w912, f="VList") -> (s? t:f=w908:string)
          n541 = Select(t=38, s=w916, f=37) -> (s? t:f=w913:i32)
          n542 = Build Array(w918, w908) -> (w917:string[])
        }
        n543 = call "VIH Utility - UI - Drag and Drop Supporter (w Symbol Indices).vi"("Cmd"=enum16{"make symbols", "test D'n'D"}."make symbols", "Item Symbols"=w897) -> ("Item Symbols out"=w896:i32[])  [unwired: 7 in, 2 out]
        n544 = control-ref of="CtrlRule List"() -> (w894:refnum<vi>)
        n545 = property on="CtrlRule List" class="MCListbox (strict)"("ItemNames"=w898, "ItemSyms"=w896) -> (error out=w887:errorcluster)  [unwired: 2 in, 1 out]
        n546 = case shown="\"INIT\"" w888 {
          tunnel: w891 -> [_ w907]
          tunnel: w890 -> [w904 w906]
          tunnel: [w904 w905] -> w889
          tunnel: w887 -> [_ _]
          frame Default {
          }
          frame "INIT" {
            n547 = call "VIH UI - Coerce List Value.vi"("# elements"=w907, "Indices in"=w906) -> ("Indices out"=w905:i32[])  [unwired: 9 in]
            n548 = property on="CtrlRule List" class="MCListbox (strict)"("Value"=w905) -> ()  [unwired: 2 in, 2 out]
          }
        }
        n549 = Index Array(array=w889) -> (element=w893:i32)  [unwired: 1 in]
        n550 = call "VIH Utility - UI - Make Row Visible (MC Listbox).vi"("Row"=w893, "MC Listbox Refnum"=w894) -> ()  [unwired: 8 in, 2 out]
      }
      frame "------------------------------ 3" {
      }
      frame "Apply: Product Info" {
        n551 = Unbundle(w929) -> ("Array out"=w928:string[], "Item Rule out"=w926:T29)
        n552 = in-place {
          n553 = in-place-cluster #1(w926) -> ("ProductInfoMode"=w930:T2)  [unwired: 1 out]
          n554 = Type Cast(type=w930, x="ProductInfoMode") -> (*(type *) &x=w931:T2)
          n555 = in-place-cluster #1("ProductInfoMode"=w931, "ProductInfoText"="ProductInfoText") -> (w925:T29)
        }
        n556 = Concatenate Strings("Globals = Set;\n\nUpdate: Product Info;" ("string"), w923) -> (w922:string)
        n557 = Bundle("Array out"=w928, "Item Rule out"=w925) -> (w927:T32)  [unwired: 1 in]
      }
      frame "Apply: General" {
        n558 = Unbundle(w940) -> ("Array out"=w939:string[], "Item Rule out"=w937:T29)
        n559 = in-place {
          n560 = in-place-cluster #2(w937) -> ()  [unwired: 6 out]
          n561 = Greater Than 0?(x="Custom_OutFile") -> (x > 0?=w947:bool)
          n562 = call "VIH Utility - FILE - Make Valid Filename.vi"("comply to CHM (F)"=TRUE, "File Name in"="Out File Name") -> ("File Name out"=w945:string)  [unwired: 9 in]
          n563 = Select(t=w945, s=w947, f="") -> (s? t:f=w944:string)
          n564 = in-place-cluster #2("OutName"=w944, "BuildHelp"="BuildHelp", "Flags.Override CSS Files"="Override_CSS Files", "Flags.Override JS Files"="Override_JS Files", "Flags.Override Ctl Rules"="Override_Ctl Rules", "%Comments"="Comments") -> (w936:T29)
        }
        n565 = Concatenate Strings("Globals = Set;\n\nUpdate: General;" ("string"), w941) -> (w935:string)
        n566 = Bundle("Array out"=w939, "Item Rule out"=w936) -> (w938:T32)  [unwired: 1 in]
      }
      frame "Apply: Target Paths" {
        n567 = Unbundle(w961) -> ("Array out"=w960:string[], "Item Rule out"=w958:T29)
        n568 = in-place {
          n569 = in-place-cluster #3(w958) -> ()  [unwired: 4 out]
          n570 = call "VIH Constant - Default Path Keyword.vi"() -> ("<default> path"=w962:path)  [unwired: 11 in]
          n571 = Greater Than 0?(x="Custom_Image Dir") -> (x > 0?=w977:bool)
          n572 = Greater Than 0?(x="Custom_HTML Dir") -> (x > 0?=w978:bool)
          n573 = Greater Than 0?(x="Custom_CSS Dir") -> (x > 0?=w976:bool)
          n574 = Greater Than 0?(x="Custom_JS Dir") -> (x > 0?=w975:bool)
          n575 = Select(t="Dst_Image Dir", s=w977, f=w962) -> (s? t:f=w965:path)
          n576 = Select(t="Dst_HTML Dir", s=w978, f=w962) -> (s? t:f=w966:path)
          n577 = Select(t="Dst_CSS Dir", s=w976, f=w962) -> (s? t:f=w964:path)
          n578 = Select(t="Dst_JS Dir", s=w975, f=w962) -> (s? t:f=w963:path)
          n579 = in-place-cluster #3("Target Paths.HTML Dir"=w966, "Target Paths.Image Dir"=w965, "Target Paths.CSS Dir"=w964, "Target Paths.JS Dir"=w963) -> (w957:T29)
        }
        n580 = Concatenate Strings("Globals = Set;\n\nUpdate: Target Paths;" ("string"), w955) -> (w954:string)
        n581 = Bundle("Array out"=w960, "Item Rule out"=w957) -> (w959:T32)  [unwired: 1 in]
      }
      frame "Apply: Templates" {
        n582 = Unbundle(w986) -> ("Array out"=w985:string[], "Item Rule out"=w983:T29)
        n583 = in-place {
          n584 = in-place-cluster #4(w983) -> ()  [unwired: 1 out]
          n585 = call "VIH Project - Container - Project File Path.vi"() -> ("Project File Path"=w988:path)  [unwired: 9 in, 2 out]
          n586 = call "VIH Constant - Default Path Keyword.vi"() -> ("<default> path"=w992:path)  [unwired: 11 in]
          n587 = Strip Path(path=w988) -> (stripped path=w987:path)  [unwired: 1 out]
          n588 = Greater Than 0?(x="Custom_Template") -> (x > 0?=w993:bool)
          n589 = call "VIH HelpGen - FILE - Build Absolute Path.vi"("Root Path"=w987, "Allow Empty Path (T)"=TRUE, "Path in"="Src_Template") -> ("Path out"=w989:path)  [unwired: 8 in]
          n590 = Select(t=w989, s=w993, f=w992) -> (s? t:f=w994:path)
          n591 = in-place-cluster #4("Source Paths.Html Template"=w994) -> (w982:T29)
        }
        n592 = Concatenate Strings("Globals = Set;\n\nUpdate: Templates;" ("string"), w980) -> (w979:string)
        n593 = Bundle("Array out"=w985, "Item Rule out"=w982) -> (w984:T32)  [unwired: 1 in]
      }
      frame "Apply: Item Rules" {
        n594 = Unbundle(w1003) -> ("Array out"=w1002:string[], "Item Rule out"=w1000:T29)
        n595 = in-place {
          n596 = in-place-cluster #5(w1000) -> ()  [unwired: 8 out]
          n597 = in-place-cluster #5("DscrMode"="VIDscrMode", "Description"="VIDescription", "Ctl_DscrMode"="Ctl_DscrMode", "Ctl_ClustMembers"="Ctl_ClustMembers", "Ctl_EnumValues"="Ctl_EnumValues", "MenuItemIcons"="MenuItemIcons", "DetailsMode"="VIDetailsMode", "DetailsText"="VIDetails") -> (w999:T29)
        }
        n598 = Concatenate Strings("Globals = Set;\n\nUpdate: Item Rules;" ("string"), w997) -> (w996:string)
        n599 = Bundle("Array out"=w1002, "Item Rule out"=w999) -> (w1001:T32)  [unwired: 1 in]
      }
      frame "------------------------------ 4" {
      }
      frame "CtrlRule: Update Controls" {
        n600 = property on="CtrlRule List" class="MCListbox (strict)"() -> ("DisabledEnum"=w1017:T11)  [unwired: 2 in, 2 out]
        n601 = Equal To 0?(x=w1017) -> (x = 0?=w1016:bool)
        n602 = case shown="\"INIT\"" w1014 {
          frame Default {
          }
          frame "INIT" {
            n603 = control-ref of="CtrlRule_CtrlID"() -> (w1034:refnum<vi>)
            n604 = control-ref of="CtrlRule_CustomName"() -> (w1033:refnum<vi>)
            n605 = control-ref of="CtrlRule_Description"() -> (w1032:refnum<vi>)
            n606 = Build Array(w1034, w1033, w1032) -> (w1031:refnum<vi>[])
            n607 = for {
              tunnel: w1031 -> [w1035] mode=indexing
              n608 = property on="Property Node" class="Str"(reference=w1035, "Text.Selection"=T12 {"Selection Start"=0, "Selection End"=0}) -> ()  [unwired: 1 in, 2 out]
            }
          }
        }
        n609 = case shown="True" w1016 {
          tunnel: w1029 -> [_ w1053]
          tunnel: [_ w1050] -> w1028
          tunnel: [_ w1049] -> w1027
          tunnel: [_ w1048] -> w1026
          tunnel: [_ w1047] -> w1025
          tunnel: [_ w1046] -> w1024
          tunnel: [_ w1045] -> w1023
          tunnel: [w1037 w1044] -> w1022
          tunnel: w1021 -> [_ w1043]
          tunnel: [w1037 w1041] -> w1020
          tunnel: [_ w1039] -> w1019
          tunnel: [w1037 w1038] -> w1018
          tunnel: [w1037 _] -> w1015
          frame False {
            w1037 = u8 2
          }
          frame True {
            n610 = Unbundle(w1053) -> ("Item Rule out"=w1052:T29)  [unwired: 1 out]
            n611 = Unbundle By Name(w1052) -> ("Control Rules"=w1051:T19[])
            n612 = Index Array(array=w1043) -> (element=w1040:i32)  [unwired: 1 in]
            n613 = Array Size(array=w1043) -> (size(s)=w1042:i32)
            n614 = case shown="..0" w1042 {
              tunnel: w1040 -> [_ w1067 _]
              tunnel: w1051 -> [_ w1066 _]
              tunnel: [_ w1064 _] -> w1050
              tunnel: [_ w1063 _] -> w1049
              tunnel: [_ w1059 _] -> w1048
              tunnel: [_ w1062 _] -> w1047
              tunnel: [_ w1061 _] -> w1046
              tunnel: [_ w1060 _] -> w1045
              tunnel: [w1054 _ w1068] -> w1038
              tunnel: [w1054 w1057 w1068] -> w1044
              tunnel: [w1054 _ _] -> w1041
              tunnel: [_ w1055 _] -> w1039
              frame ..0 {
                w1054 = u8 2
              }
              frame 1 {
                n615 = Index Array(array=w1066, index=w1067) -> (element=w1065:T19)
                n616 = Unbundle By Name(w1065) -> ("CtrlID"=w1064:string, "CustomRule"=w1063:bool, "DscrMode"=w1059:T7, "Description"=w1062:string, "ClusterMembers"=w1061:T2, "EnumValues"=w1060:T2, "CustomName"=w1055:string)
                n617 = Equal?(x=VIH_HelpGen_Typedef_-_Enum_-_Description_Mode."Custom", y=w1059) -> (x = y?=w1056:bool)
                n618 = call "VIH Utility - UI - Boolean to Control Disable Status.vi"("Status in"=w1056) -> ("Control Disable if False"=w1057:u8)  [unwired: 3 in, 1 out]
              }
              frame 2.. {
                w1068 = u8 2
              }
            }
          }
        }
        n619 = property on="%CtrlRule_Add" class="Bool"("DisabledEnum"=w1015) -> ()  [unwired: 2 in, 2 out]
        n620 = property on="%CtrlRule_Copy" class="Bool"("DisabledEnum"=w1020) -> ()  [unwired: 2 in, 2 out]
        n621 = property on="CtrlRule_CtrlID" class="Str"("DisabledEnum"=w1018, "Value"=w1028) -> ()  [unwired: 2 in, 2 out]
        n622 = property on="CtrlRule_DscrMode" class="Enum (strict)"("DisabledEnum"=w1018, "Value"=w1026) -> ()  [unwired: 2 in, 2 out]
        n623 = property on="CtrlRule_ClusterMembers" class="Enum (strict)"("DisabledEnum"=w1018, "Value"=w1024) -> ()  [unwired: 2 in, 2 out]
        n624 = property on="CtrlRule_CustomName" class="Str"("DisabledEnum"=w1018, "Value"=w1019) -> ()  [unwired: 2 in, 2 out]
        n625 = property on="CtrlRule_CustomRule" class="Bool (strict)"("DisabledEnum"=w1018, "Value"=w1027) -> ()  [unwired: 2 in, 2 out]
        n626 = property on="CtrlRule_Description" class="Str"("DisabledEnum"=w1022, "Value"=w1025) -> ()  [unwired: 2 in, 2 out]
        n627 = property on="CtrlRule_EnumValues" class="Enum (strict)"("DisabledEnum"=w1018, "Value"=w1023) -> ()  [unwired: 2 in, 2 out]
        n628 = property on="%CtrlRule_Remove" class="Bool"("DisabledEnum"=w1020) -> ()  [unwired: 2 in, 2 out]
        n629 = property on="%CtrlRule_Import" class="Bool"("DisabledEnum"=w1015) -> ()  [unwired: 2 in, 2 out]
        n630 = property on="%CtrlRule_Edit_Enum" class="Bool"("DisabledEnum"=w1018) -> ()  [unwired: 2 in, 2 out]
      }
      frame "CtrlRule: Add" {
        n631 = Unbundle(w1079) -> ("Item Rule out"=w1081:T29)  [unwired: 1 out]
        n632 = Array Size(array=w1071) -> (size(s)=w1075:i32)
        n633 = Array Max & Min(array=w1071) -> (max value=w1073:i32)  [unwired: 3 out]
        n634 = Less Or Equal To 0?(x=w1075) -> (x <= 0?=w1074:bool)
        n635 = Select(t=-1, s=w1074, f=w1073) -> (s? t:f=w1070:i32)
        n636 = Increment(x=w1070) -> (x+1=w1069:i32)
        n637 = in-place {
          in-place-border: w1069 -> [w1083]
          n638 = in-place-cluster #6(w1081) -> ("Control Rules"=w1091:T19[])
          n639 = Array Size(array=w1091) -> (size(s)=w1092:i32)
          n640 = Index Array(array=w1091, index=-1 ("f")) -> (element=w1090:T19)
          n641 = In Range and Coerce(upper limit=w1092, x=w1083, lower limit=0) -> (coerced(x)=w1088:i32)  [unwired: 1 out]
          n642 = Bundle By Name(cluster=w1090, "CtrlID"="<Control Name>", "CustomRule"=TRUE) -> (w1089:T19)
          n643 = Build Array(w1088) -> (w1087:i32[])
          n644 = local write "CtrlRule List"(w1087) -> ()
          n645 = Insert Into Array(array=w1091, index=w1088, new element=w1089) -> (w1094:T19[])
          n646 = in-place-cluster #6("Control Rules"=w1094) -> (w1080:T29)
        }
        n647 = Concatenate Strings("Globals = Set;\n\nUpdate: Control Rules;\nCtrlRule: Update Controls = INIT;" ("string"), w1082) -> (w1077:string)
        n648 = Bundle(cluster=w1079, "Item Rule out"=w1080) -> (w1078:T32)  [unwired: 1 in]
      }
      frame "CtrlRule: Import" {
        n649 = case shown="\"VI\", Default" w1100 {
          tunnel: [w1117 w1124] -> w1101
          tunnel: [TRUE w1123] -> w1099
          tunnel: w1098 -> [w1110 _]
          tunnel: [w1107 -1 ("t")] -> w1097
          tunnel: w1096 -> [_ _]
          tunnel: w1095 -> [_ w1120]
          frame "CB", "Clipboard" {
            n650 = invoke class="App" method="Clipboard.Read"() -> ("Read Clipbrd"=w1116:string)  [unwired: 3 in, 2 out]
            n651 = Array Size(array=w1110) -> (size(s)=w1113:i32)
            n652 = Array Max & Min(array=w1110) -> (max value=w1108:i32)  [unwired: 3 out]
            n653 = Less Or Equal To 0?(x=w1113) -> (x <= 0?=w1112:bool)
            n654 = Select(t=-1, s=w1112, f=w1108) -> (s? t:f=w1109:i32)
            n655 = call "VIH XML - Control Rules to-from XML String.vi"("cmd (check)"=enum16{"check", "parse", "format"}."parse", "XML in"=w1116) -> ("Control Rules out"=w1117:T19[])  [unwired: 6 in, 3 out]
            n656 = Increment(x=w1109) -> (x+1=w1107:i32)
          }
          frame "VI", Default {
            n657 = Unbundle(w1120) -> ("Array out"=w1119:string[])  [unwired: 1 out]
            n658 = Index Array(array=w1119) -> (element=w1121:string)  [unwired: 1 in]
            n659 = call "VIH Project Tree - Item Tag - Parse.vi"("Tree Item Tag"=w1121) -> ("Item File Path"=w1118:path)  [unwired: 8 in, 2 out]
            n660 = call "VIH Dialog - VI Terminals.vi"("VI Path"=w1118) -> ("OK out"=w1123:bool, "Ctrl Rules"=w1124:T19[])  [unwired: 7 in, 2 out]
          }
        }
        n661 = Empty Array?(array=w1101) -> (empty?=w1102:bool)
        n662 = case shown="False" w1102 {
          tunnel: w1095 -> [w1129 w1138]
          tunnel: [w1128 w1138] -> w1104
          tunnel: ["Globals = Set;\n\nUpdate: Control Rules;\nCtrlRule: Update Controls = INIT;" ("string") _] -> w1103
          tunnel: w1101 -> [w1126 _]
          tunnel: w1099 -> [_ w1137]
          tunnel: w1097 -> [w1125 _]
          frame False {
            n663 = Unbundle(w1129) -> ("Item Rule out"=w1131:T29)  [unwired: 1 out]
            n664 = in-place {
              in-place-border: w1126 -> [w1134]
              in-place-border: w1125 -> [w1132]
              n665 = in-place-cluster #7(w1131) -> ("Control Rules"=w1136:T19[])
              n666 = call "VIH UI - Append Control Rules.vi"("Position Index (-1)"=w1132, "Ctrl Rules (new)"=w1134, "Ctrl Rules (existing)"=w1136) -> ("Indices"=w1133:i32[], "Ctrl Rules out"=w1135:T19[])  [unwired: 7 in]
              n667 = in-place-cluster #7("Control Rules"=w1135) -> (w1130:T29)
              n668 = property on="CtrlRule List" class="MCListbox (strict)"("Value"=w1133) -> ()  [unwired: 2 in, 2 out]
            }
            n669 = Bundle(cluster=w1129, "Item Rule out"=w1130) -> (w1128:T32)  [unwired: 1 in]
          }
          frame True {
            n670 = case shown="True" w1137 {
              frame False {
              }
              frame True {
                n671 = call <vilib>:"Beep.vi"() -> ()  [unwired: 12 in]
              }
            }
          }
        }
        n672 = Concatenate Strings(w1103, w1106) -> (w1105:string)
      }
      frame "CtrlRule: Export" {
        n673 = Unbundle(w1145) -> ("Item Rule out"=w1147:T29)  [unwired: 1 out]
        n674 = Unbundle By Name(w1147) -> ("Control Rules"=w1144:T19[])
        n675 = for {
          tunnel: w1146 -> [w1151] mode=indexing
          tunnel: w1144 -> [w1150]
          tunnel: [w1149] -> w1139 mode=indexing
          n676 = Index Array(array=w1150, index=w1151) -> (element=w1149:T19)
        }
        n677 = call "VIH XML - Control Rules to-from XML String.vi"("cmd (check)"=enum16{"check", "parse", "format"}."format", "Control Rules in"=w1139) -> ("error out"=w1142:errorcluster, "XML out"=w1141:string)  [unwired: 6 in, 2 out]
        n678 = invoke class="App" method="Clipboard.Write"(error in=w1142, "Param 0"=w1141) -> (error out=w1140:errorcluster)  [unwired: 2 in, 3 out]
        n679 = call <vilib>:"Simple Error Handler.vi"("error in (no error)"=w1140) -> ()  [unwired: 4 in, 5 out]
      }
      frame "CtrlRule: Remove" {
        n680 = Unbundle(w1157) -> ("Item Rule out"=w1159:T29)  [unwired: 1 out]
        n681 = in-place {
          in-place-border: w1153 -> [w1164]
          in-place-border: [w1161] -> w1152
          n682 = in-place-cluster #8(w1159) -> ("Control Rules"=w1163:T19[])
          n683 = Sort 1D Array(array=w1164) -> (sorted array=w1165:i32[])
          n684 = Reverse 1D Array(array=w1165) -> (reversed array=w1174:i32[])
          n685 = for {
            tunnel: w1174 -> [w1175] mode=indexing
            shift-right: [w1177] -> w1162
            shift-left: w1163 -> [w1176]
            n686 = Delete From Array(array=w1176, index=w1175) -> (array with subset deleted=w1177:T19[])  [unwired: 1 in, 1 out]
          }
          n687 = Index Array(array=w1165) -> (element=w1173:i32)  [unwired: 1 in]
          n688 = Array Size(array=w1162) -> (size(s)=w1171:i32)
          n689 = Decrement(x=w1171) -> (x-1=w1166:i32)
          n690 = In Range and Coerce(upper limit=w1166, x=w1173, lower limit=0) -> (coerced(x)=w1169:i32)  [unwired: 1 out]
          n691 = Less Than 0?(x=w1166) -> (x < 0?=w1170:bool)
          n692 = Build Array(w1169) -> (w1168:i32[])
          n693 = Select(t=i32[] [] ("CSS List"), s=w1170, f=w1168) -> (s? t:f=w1161:i32[])
          n694 = in-place-cluster #8("Control Rules"=w1162) -> (w1158:T29)
        }
        n695 = local write "CtrlRule List"(w1152) -> ()
        n696 = Bundle(cluster=w1157, "Item Rule out"=w1158) -> (w1156:T32)  [unwired: 1 in]
        n697 = Concatenate Strings("Globals = Set;\n\nUpdate: Control Rules;\nCtrlRule: Update Controls = INIT;" ("string"), w1160) -> (w1155:string)
      }
      frame "CtrlRule: Dragged" {
        n698 = Unbundle(w1181) -> ("Item Rule out"=w1183:T29)  [unwired: 1 out]
        n699 = in-place {
          n700 = in-place-cluster #9(w1183) -> ("Control Rules"=w1186:T19[])
          n701 = property on="CtrlRule List" class="MCListbox (strict)"() -> ("ItemSyms"=w1189:i32[])  [unwired: 2 in, 2 out]
          n702 = call "VIH Utility - UI - Drag and Drop Supporter (w Symbol Indices).vi"("Cmd"=enum16{"make symbols", "test D'n'D"}."test D'n'D", "Item Symbols"=w1189) -> ("indices"=w1187:i32[])  [unwired: 7 in, 2 out]
          n703 = for {
            tunnel: w1187 -> [w1192] mode=indexing
            tunnel: w1186 -> [w1191]
            tunnel: [w1190] -> w1185 mode=indexing
            n704 = Index Array(array=w1191, index=w1192) -> (element=w1190:T19)
          }
          n705 = in-place-cluster #9("Control Rules"=w1185) -> (w1182:T29)
        }
        n706 = Concatenate Strings("Globals = Set;\n\nUpdate: Control Rules;\nCtrlRule: Update Controls = INIT;" ("string"), w1184) -> (w1179:string)
        n707 = Bundle(cluster=w1181, "Item Rule out"=w1182) -> (w1180:T32)  [unwired: 1 in]
      }
      frame "CtrlRule: Apply" {
        n708 = Unbundle(w1198) -> ("Item Rule out"=w1200:T29)  [unwired: 1 out]
        n709 = Decimal String To Number(string=w1193, default (0L)=-1 ("default (0 I32)")) -> (number=w1196:i32)  [unwired: 1 in, 1 out]
        n710 = in-place {
          in-place-border: w1196 -> [w1205]
          n711 = in-place-cluster #10(w1200) -> ("Control Rules"=w1204:T19[])
          n712 = in-place {
            n713 = in-place-array #11(w1204, w1205) -> (w1219:T19)
            n714 = call <vilib>:"Trim Whitespace.vi"("string"="CtrlRule_CtrlID") -> ("trimmed string"=w1209:string)  [unwired: 1 in]
            n715 = call <vilib>:"Trim Whitespace.vi"("string"="CtrlRule_CustomName") -> ("trimmed string"=w1207:string)  [unwired: 1 in]
            n716 = Empty String/Path?(string/path=w1209) -> (empty?=w1213:bool)
            n717 = Select(t="<Control ID>", s=w1213, f=w1209) -> (s? t:f=w1211:string)
            n718 = Bundle By Name(cluster=w1219, "CtrlID"=w1211, "CustomRule"="CtrlRule_CustomRule", "DscrMode"="CtrlRule_DscrMode", "Description"="CtrlRule_Description", "ClusterMembers"="CtrlRule_ClustMembers", "EnumValues"="CtrlRule_EnumValues", "CustomName"=w1207) -> (w1218:T19)
            n719 = in-place-array #11(w1218) -> (w1203:T19[])  [unwired: 1 out]
          }
          n720 = in-place-cluster #10("Control Rules"=w1203) -> (w1199:T29)
        }
        n721 = Concatenate Strings("Globals = Set;\n\nUpdate: Control Rules;\nCtrlRule: Update Controls;" ("string"), w1202) -> (w1195:string)
        n722 = Bundle(cluster=w1198, "Item Rule out"=w1199) -> (w1197:T32)  [unwired: 1 in]
      }
      frame "CtrlRule: Enable" {
        n723 = Unbundle(w1233) -> ("Item Rule out"=w1235:T29)  [unwired: 1 out]
        n724 = Match Pattern(string=w1228, regular expression="\\?") -> (before substring=w1227:string, after substring=w1225:string)  [unwired: 1 in, 2 out]
        n725 = Decimal String To Number(string=w1227) -> (number=w1224:i32)  [unwired: 2 in, 1 out]
        n726 = call "VIH Utility - STR - String to 1D Str Array.vi"("delimiter ('\\n')"="," ("delimiter ('\\n')"), "String in"=w1225) -> ("Array out"=w1222:string[])  [unwired: 5 in]
        n727 = Not Equal To 0?(x=w1224) -> (x != 0?=w1223:bool)
        n728 = Decimal String To Number(string=w1222, default (0L)=-1 ("default (0 I32)")) -> (number=w1220:i32[])  [unwired: 1 in, 1 out]
        n729 = in-place {
          in-place-border: w1223 -> [w1238]
          in-place-border: w1220 -> [w1237]
          n730 = in-place-cluster #12(w1235) -> ("Control Rules"=w1240:T19[])
          n731 = for {
            tunnel: w1237 -> [w1244] mode=indexing
            shift-right: [w1242] -> w1239
            shift-left: w1240 -> [w1243]
            tunnel: w1238 -> [w1241]
            n732 = in-place {
              in-place-border: w1241 -> [w1245]
              n733 = in-place-array #13(w1243, w1244) -> (w1247:T19)
              n734 = Bundle By Name(cluster=w1247, "CustomRule"=w1245) -> (w1246:T19)
              n735 = in-place-array #13(w1246) -> (w1242:T19[])  [unwired: 1 out]
            }
          }
          n736 = in-place-cluster #12("Control Rules"=w1239) -> (w1234:T29)
        }
        n737 = Concatenate Strings("Globals = Set;\n\nUpdate: Control Rules;\nCtrlRule: Update Controls;" ("string"), w1236) -> (w1231:string)
        n738 = Bundle(cluster=w1233, "Item Rule out"=w1234) -> (w1232:T32)  [unwired: 1 in]
      }
      frame "CtrlRule: Edit Enum Values" {
        n739 = Unbundle(w1256) -> ("Array out"=w1249:string[], "Item Rule out"=w1258:T29)
        n740 = Decimal String To Number(string=w1251, default (0L)=-1 ("default (0 I32)")) -> (number=w1254:i32)  [unwired: 1 in, 1 out]
        n741 = Index Array(array=w1249) -> (element=w1248:string)  [unwired: 1 in]
        n742 = in-place {
          in-place-border: w1254 -> [w1265]
          in-place-border: w1250 -> [w1262]
          in-place-border: w1248 -> [w1261]
          n743 = in-place-cluster #14(w1258) -> ("Control Rules"=w1264:T19[])
          n744 = in-place {
            in-place-border: w1262 -> [w1269]
            in-place-border: w1261 -> [w1268]
            n745 = in-place-array #15(w1264, w1265) -> (w1273:T19)
            n746 = call "VIH Project Tree - Item Tag - Parse.vi"("Tree Item Tag"=w1268) -> ("Item File Path"=w1266:path)  [unwired: 8 in, 2 out]
            n747 = Unbundle By Name(w1273) -> ("EnumValDscr"=w1271:T20[], "CtrlID"=w1267:string)
            n748 = call "VIH Dialog - Enum Values.vi"("VI Path"=w1266, "Control ID"=w1267, "EnumValDefs in"=w1271, "Project Tree"=w1269) -> ("OK out"=w1274:bool, "EnumValDefs out"=w1270:T20[])  [unwired: 6 in]
            n749 = case shown="True" w1274 {
              tunnel: [w1275 w1278] -> w1272
              tunnel: w1273 -> [w1275 w1277]
              tunnel: w1270 -> [_ w1276]
              frame False {
              }
              frame True {
                n750 = Bundle By Name(cluster=w1277, "EnumValDscr"=w1276) -> (w1278:T19)
              }
            }
            n751 = in-place-array #15(w1272) -> (w1263:T19[])  [unwired: 1 out]
          }
          n752 = in-place-cluster #14("Control Rules"=w1263) -> (w1257:T29)
        }
        n753 = Concatenate Strings("Globals = Set;\n\nUpdate: Control Rules;\nCtrlRule: Update Controls;" ("string"), w1260) -> (w1253:string)
        n754 = Bundle(cluster=w1256, "Item Rule out"=w1257) -> (w1255:T32)  [unwired: 1 in]
      }
      frame "------------------------------ 5" {
      }
      frame "CSS List: Update Controls" {
        n755 = property on="CSS List" class="MCListbox (strict)"() -> ("DisabledEnum"=w1283:T11)  [unwired: 2 in, 2 out]
        n756 = Equal To 0?(x=w1283) -> (x = 0?=w1282:bool)
        n757 = case shown="True" w1282 {
          tunnel: [w1289 w1296] -> w1287
          tunnel: w1286 -> [_ w1295]
          tunnel: w1285 -> [_ w1292]
          tunnel: [_ w1290] -> w1284
          tunnel: [w1289 _] -> w1281
          frame False {
            w1289 = u8 2 ("Control Disable if True")
          }
          frame True {
            n758 = Unbundle(w1295) -> ("Item Rule out"=w1294:T29)  [unwired: 1 out]
            n759 = Unbundle By Name(w1294) -> ("Source Paths.CSS Files"=w1293:path[])
            n760 = Index Array(array=w1292) -> (element=w1291:i32)  [unwired: 1 in]
            n761 = Empty Array?(array=w1292) -> (empty?=w1297:bool)
            n762 = call "VIH Utility - UI - Boolean to Control Disable Status.vi"("Status in"=w1297) -> ("Control Disable if True"=w1296:u8)  [unwired: 3 in, 1 out]
            n763 = Index Array(array=w1293, index=w1291) -> (element=w1290:path)
          }
        }
        "CSS File" <- w1284
        n764 = property on="%CSS List_Add" class="Bool"("DisabledEnum"=w1281) -> ()  [unwired: 2 in, 2 out]
        n765 = property on="%CSS List_Remove" class="Bool"("DisabledEnum"=w1287) -> ()  [unwired: 2 in, 2 out]
      }
      frame "CSS List: Make Selection Visible" {
        n766 = control-ref of="CSS List"() -> (w1304:refnum<vi>)
        n767 = property class="MCListbox (strict)"(reference=w1304) -> (reference out=w1303:refnum<vi>, "Value"=w1302:i32[])  [unwired: 1 in, 1 out]
        n768 = Empty Array?(array=w1302) -> (empty?=w1301:bool)
        n769 = Index Array(array=w1302) -> (element=w1300:i32)  [unwired: 1 in]
        n770 = Select(t=-1, s=w1301, f=w1300) -> (s? t:f=w1298:i32)
        n771 = call "VIH Utility - UI - Make Row Visible (MC Listbox).vi"("Row"=w1298, "MC Listbox Refnum"=w1303) -> ()  [unwired: 8 in, 2 out]
      }
      frame "CSS List: Add" {
        n772 = Array Size(array=w1310) -> (size(s)=w1308:i32)
        n773 = Unbundle(w1320) -> ("Item Rule out"=w1313:T29)  [unwired: 1 out]
        n774 = Array Max & Min(array=w1310) -> (max value=w1312:i32)  [unwired: 3 out]
        n775 = Less Or Equal To 0?(x=w1308) -> (x <= 0?=w1309:bool)
        n776 = Select(t=-1, s=w1309, f=w1312) -> (s? t:f=w1311:i32)
        n777 = call "File Dialog"("pattern (all files)"="*.css") -> ("selected paths"=w1316:path[], "error out"=w1317:errorcluster)  [unwired: 11 in, 2 out]
        n778 = case shown="No Error" w1317 {
          tunnel: w1313 -> [w1327 w1341]
          tunnel: [w1326 w1341] -> w1321
          tunnel: w1311 -> [w1325 _]
          tunnel: w1316 -> [w1324 _]
          tunnel: ["Globals = Set;\n\nUpdate: CSS List;\nCSS List: Make Selection Visible;\nCSS List: Update Controls;" ("string") _] -> w1314
          frame No Error {
            n779 = in-place {
              in-place-border: w1325 -> [w1333]
              in-place-border: w1324 -> [w1328]
              n780 = in-place-cluster #16(w1327) -> ("Source Paths.CSS Files"=w1334:path[])
              n781 = Increment(x=w1333) -> (x+1=w1332:i32)
              n782 = Array Size(array=w1334) -> (size(s)=w1335:i32)
              n783 = In Range and Coerce(upper limit=w1335, x=w1332, lower limit=0) -> (coerced(x)=w1331:i32)  [unwired: 1 out]
              n784 = Array Size(array=w1328) -> (size(s)=w1329:i32)
              n785 = for {
                N: w1329 -> [_]
                tunnel: w1331 -> [w1339]
                tunnel: [w1338] -> w1330 mode=indexing
                i -> [w1340]
                n786 = Add(x=w1339, y=w1340) -> (x+y=w1338:i32)
              }
              n787 = Insert Into Array(array=w1334, index=w1331, new element=w1328) -> (w1337:path[])
              n788 = in-place-cluster #16("Source Paths.CSS Files"=w1337) -> (w1326:T29)
              n789 = local write "CSS List"(w1330) -> ()
            }
          }
          frame Error {
          }
        }
        n790 = Concatenate Strings(w1314, w1322) -> (w1318:string)
        n791 = Bundle(cluster=w1320, "Item Rule out"=w1321) -> (w1319:T32)  [unwired: 1 in]
      }
      frame "CSS List: Remove" {
        n792 = Unbundle(w1346) -> ("Item Rule out"=w1348:T29)  [unwired: 1 out]
        n793 = in-place {
          in-place-border: w1342 -> [w1362]
          n794 = in-place-cluster #17(w1348) -> ("Source Paths.CSS Files"=w1363:path[])
          n795 = Sort 1D Array(array=w1362) -> (sorted array=w1352:i32[])
          n796 = Reverse 1D Array(array=w1352) -> (reversed array=w1361:i32[])
          n797 = for {
            tunnel: w1361 -> [w1364] mode=indexing
            shift-right: [w1366] -> w1351
            shift-left: w1363 -> [w1365]
            n798 = Delete From Array(array=w1365, index=w1364) -> (array with subset deleted=w1366:path[])  [unwired: 1 in, 1 out]
          }
          n799 = Index Array(array=w1352) -> (element=w1360:i32)  [unwired: 1 in]
          n800 = Array Size(array=w1351) -> (size(s)=w1358:i32)
          n801 = Decrement(x=w1358) -> (x-1=w1353:i32)
          n802 = In Range and Coerce(upper limit=w1353, x=w1360, lower limit=0) -> (coerced(x)=w1356:i32)  [unwired: 1 out]
          n803 = Less Than 0?(x=w1353) -> (x < 0?=w1357:bool)
          n804 = Build Array(w1356) -> (w1355:i32[])
          n805 = in-place-cluster #17("Source Paths.CSS Files"=w1351) -> (w1347:T29)
          n806 = Select(t=i32[] [] ("CSS List"), s=w1357, f=w1355) -> (s? t:f=w1350:i32[])
          n807 = local write "CSS List"(w1350) -> ()
        }
        n808 = Concatenate Strings("Globals = Set;\n\nUpdate: CSS List;\nCSS List: Make Selection Visible;\nCSS List: Update Controls;" ("string"), w1349) -> (w1344:string)
        n809 = Bundle(cluster=w1346, "Item Rule out"=w1347) -> (w1345:T32)  [unwired: 1 in]
      }
      frame "CSS List: Dragged" {
        n810 = Unbundle(w1370) -> ("Item Rule out"=w1372:T29)  [unwired: 1 out]
        n811 = in-place {
          n812 = in-place-cluster #18(w1372) -> ("Source Paths.CSS Files"=w1375:path[])
          n813 = property on="CSS List" class="MCListbox (strict)"() -> ("ItemSyms"=w1378:i32[])  [unwired: 2 in, 2 out]
          n814 = call "VIH Utility - UI - Drag and Drop Supporter (w Symbol Indices).vi"("Cmd"=enum16{"make symbols", "test D'n'D"}."test D'n'D", "Item Symbols"=w1378) -> ("indices"=w1376:i32[])  [unwired: 7 in, 2 out]
          n815 = for {
            tunnel: w1376 -> [w1381] mode=indexing
            tunnel: w1375 -> [w1380]
            tunnel: [w1379] -> w1374 mode=indexing
            n816 = Index Array(array=w1380, index=w1381) -> (element=w1379:path)
          }
          n817 = in-place-cluster #18("Source Paths.CSS Files"=w1374) -> (w1371:T29)
        }
        n818 = Concatenate Strings("Globals = Set;\n\nUpdate: CSS List;\n\nCSS List: Update Controls;" ("string"), w1373) -> (w1368:string)
        n819 = Bundle(cluster=w1370, "Item Rule out"=w1371) -> (w1369:T32)  [unwired: 1 in]
      }
      frame "------------------------------ 6" {
      }
      frame "JS List: Update Controls" {
        n820 = property on="JS List" class="MCListbox (strict)"() -> ("DisabledEnum"=w1386:T11)  [unwired: 2 in, 2 out]
        n821 = Equal To 0?(x=w1386) -> (x = 0?=w1385:bool)
        n822 = case shown="True" w1385 {
          tunnel: [w1392 w1399] -> w1390
          tunnel: w1389 -> [_ w1398]
          tunnel: [_ w1394] -> w1388
          tunnel: w1387 -> [_ w1393]
          tunnel: [w1392 _] -> w1384
          frame False {
            w1392 = u8 2 ("Control Disable if True")
          }
          frame True {
            n823 = Unbundle(w1398) -> ("Item Rule out"=w1397:T29)  [unwired: 1 out]
            n824 = Unbundle By Name(w1397) -> ("Source Paths.JS Files"=w1396:path[])
            n825 = Index Array(array=w1393) -> (element=w1395:i32)  [unwired: 1 in]
            n826 = Empty Array?(array=w1393) -> (empty?=w1400:bool)
            n827 = call "VIH Utility - UI - Boolean to Control Disable Status.vi"("Status in"=w1400) -> ("Control Disable if True"=w1399:u8)  [unwired: 3 in, 1 out]
            n828 = Index Array(array=w1396, index=w1395) -> (element=w1394:path)
          }
        }
        "JS File" <- w1388
        n829 = property on="%JS List_Add" class="Bool"("DisabledEnum"=w1384) -> ()  [unwired: 2 in, 2 out]
        n830 = property on="%JS List_Remove" class="Bool"("DisabledEnum"=w1390) -> ()  [unwired: 2 in, 2 out]
      }
      frame "JS List: Make Selection Visible" {
        n831 = control-ref of="JS List"() -> (w1407:refnum<vi>)
        n832 = property class="MCListbox (strict)"(reference=w1407) -> (reference out=w1406:refnum<vi>, "Value"=w1405:i32[])  [unwired: 1 in, 1 out]
        n833 = Empty Array?(array=w1405) -> (empty?=w1404:bool)
        n834 = Index Array(array=w1405) -> (element=w1403:i32)  [unwired: 1 in]
        n835 = Select(t=-1, s=w1404, f=w1403) -> (s? t:f=w1401:i32)
        n836 = call "VIH Utility - UI - Make Row Visible (MC Listbox).vi"("Row"=w1401, "MC Listbox Refnum"=w1406) -> ()  [unwired: 8 in, 2 out]
      }
      frame "JS List: Add" {
        n837 = Array Size(array=w1411) -> (size(s)=w1413:i32)
        n838 = Unbundle(w1423) -> ("Item Rule out"=w1416:T29)  [unwired: 1 out]
        n839 = Array Max & Min(array=w1411) -> (max value=w1415:i32)  [unwired: 3 out]
        n840 = Less Or Equal To 0?(x=w1413) -> (x <= 0?=w1414:bool)
        n841 = Select(t=-1, s=w1414, f=w1415) -> (s? t:f=w1412:i32)
        n842 = call "File Dialog2"("pattern (all files)"="*.js") -> ("selected paths"=w1419:path[], "error out"=w1420:errorcluster)  [unwired: 11 in, 2 out]
        n843 = case shown="No Error" w1420 {
          tunnel: w1416 -> [w1430 w1444]
          tunnel: [w1429 w1444] -> w1424
          tunnel: w1412 -> [w1428 _]
          tunnel: w1419 -> [w1427 _]
          tunnel: ["Globals = Set;\n\nUpdate: JS List;\nJS List: Make Selection Visible;\nJS List: Update Controls;" ("string") _] -> w1417
          frame No Error {
            n844 = in-place {
              in-place-border: w1428 -> [w1436]
              in-place-border: w1427 -> [w1431]
              n845 = in-place-cluster #19(w1430) -> ("Source Paths.JS Files"=w1437:path[])
              n846 = Increment(x=w1436) -> (x+1=w1435:i32)
              n847 = Array Size(array=w1437) -> (size(s)=w1438:i32)
              n848 = In Range and Coerce(upper limit=w1438, x=w1435, lower limit=0) -> (coerced(x)=w1434:i32)  [unwired: 1 out]
              n849 = Array Size(array=w1431) -> (size(s)=w1432:i32)
              n850 = for {
                N: w1432 -> [_]
                tunnel: w1434 -> [w1442]
                tunnel: [w1441] -> w1433 mode=indexing
                i -> [w1443]
                n851 = Add(x=w1442, y=w1443) -> (x+y=w1441:i32)
              }
              n852 = Insert Into Array(array=w1437, index=w1434, new element=w1431) -> (w1440:path[])
              n853 = in-place-cluster #19("Source Paths.JS Files"=w1440) -> (w1429:T29)
              n854 = local write "JS List"(w1433) -> ()
            }
          }
          frame Error {
          }
        }
        n855 = Concatenate Strings(w1417, w1425) -> (w1421:string)
        n856 = Bundle(cluster=w1423, "Item Rule out"=w1424) -> (w1422:T32)  [unwired: 1 in]
      }
      frame "JS List: Remove" {
        n857 = Unbundle(w1449) -> ("Item Rule out"=w1451:T29)  [unwired: 1 out]
        n858 = in-place {
          in-place-border: w1445 -> [w1465]
          n859 = in-place-cluster #20(w1451) -> ("Source Paths.JS Files"=w1466:path[])
          n860 = Sort 1D Array(array=w1465) -> (sorted array=w1463:i32[])
          n861 = Reverse 1D Array(array=w1463) -> (reversed array=w1464:i32[])
          n862 = for {
            tunnel: w1464 -> [w1467] mode=indexing
            shift-right: [w1469] -> w1460
            shift-left: w1466 -> [w1468]
            n863 = Delete From Array(array=w1468, index=w1467) -> (array with subset deleted=w1469:path[])  [unwired: 1 in, 1 out]
          }
          n864 = Index Array(array=w1463) -> (element=w1462:i32)  [unwired: 1 in]
          n865 = Array Size(array=w1460) -> (size(s)=w1459:i32)
          n866 = Decrement(x=w1459) -> (x-1=w1453:i32)
          n867 = In Range and Coerce(upper limit=w1453, x=w1462, lower limit=0) -> (coerced(x)=w1457:i32)  [unwired: 1 out]
          n868 = Less Than 0?(x=w1453) -> (x < 0?=w1458:bool)
          n869 = Build Array(w1457) -> (w1456:i32[])
          n870 = Select(t=i32[] [] ("CSS List"), s=w1458, f=w1456) -> (s? t:f=w1454:i32[])
          n871 = in-place-cluster #20("Source Paths.JS Files"=w1460) -> (w1450:T29)
          n872 = local write "JS List"(w1454) -> ()
        }
        n873 = Concatenate Strings("Globals = Set;\n\nUpdate: JS List;\nJS List: Make Selection Visible;\nJS List: Update Controls;" ("string"), w1452) -> (w1447:string)
        n874 = Bundle(cluster=w1449, "Item Rule out"=w1450) -> (w1448:T32)  [unwired: 1 in]
      }
      frame "JS List: Dragged" {
        n875 = Unbundle(w1473) -> ("Item Rule out"=w1475:T29)  [unwired: 1 out]
        n876 = in-place {
          n877 = in-place-cluster #21(w1475) -> ("Source Paths.JS Files"=w1478:path[])
          n878 = property on="JS List" class="MCListbox (strict)"() -> ("ItemSyms"=w1481:i32[])  [unwired: 2 in, 2 out]
          n879 = call "VIH Utility - UI - Drag and Drop Supporter (w Symbol Indices).vi"("Cmd"=enum16{"make symbols", "test D'n'D"}."test D'n'D", "Item Symbols"=w1481) -> ("indices"=w1479:i32[])  [unwired: 7 in, 2 out]
          n880 = for {
            tunnel: w1479 -> [w1484] mode=indexing
            tunnel: w1478 -> [w1483]
            tunnel: [w1482] -> w1477 mode=indexing
            n881 = Index Array(array=w1483, index=w1484) -> (element=w1482:path)
          }
          n882 = in-place-cluster #21("Source Paths.JS Files"=w1477) -> (w1474:T29)
        }
        n883 = Concatenate Strings("Globals = Set;\n\nUpdate: JS List;\n\nJS List: Update Controls;" ("string"), w1476) -> (w1471:string)
        n884 = Bundle(cluster=w1473, "Item Rule out"=w1474) -> (w1472:T32)  [unwired: 1 in]
      }
      frame "------------------------------ 7" {
      }
      frame "Control Appearance" {
        (unwired) "Control"
      }
    }
  }
  n885 = while {
    shift-right: [w1493] -> _
    shift-left: "INIT;" -> [w1496]
    tunnel: w2 -> [w1490]
    tunnel: w3 -> [w1489]
    stop <- w1491 stop-if-true
    n886 = call "VIH Utility - APP - State Queue Parser (STR).vi"("input queue"=w1496) -> ("state"=w1495:string, "remained queue"=w1492:string, "complete state specifier"=w1494:string)  [unwired: 5 in, 1 out]
    n887 = case shown="\"\"" w1495 {
      tunnel: w1494 -> [w1502 _ _ _]
      tunnel: [w1497 w1507 w1509 w1517] -> w1493
      tunnel: w1492 -> [w1498 w1507 w1509 w1516]
      tunnel: [_ _ TRUE _] -> w1491
      tunnel: w1490 -> [_ _ w1508 w1520]
      tunnel: w1489 -> [_ _ _ w1515]
      frame Default {
        n888 = property class="VI"() -> ("Name"=w1501:string)  [unwired: 2 in, 2 out]
        n889 = Format Into String(format string="%s\n(Communication Loop)\n\nUnknown state specifier:\n%s", w1501, w1502) -> (resulting string=w1505:string)  [unwired: 2 in, 1 out]
        n890 = Two Button Dialog(message=w1505, 1:"HALT" ("F button name (\"Cancel\")"), 2:"Continue" ("T button name (\"OK\")")) -> (T button?=w1499:bool)
        n891 = Select(t=w1498, s=w1499, f="HALT;") -> (s? t:f=w1497:string)
      }
      frame "INIT" {
      }
      frame "HALT" {
        n892 = Release Queue(queue=w1508) -> ()  [unwired: 2 in, 3 out]
      }
      frame "" {
        n893 = Dequeue Element(queue=w1520, timeout in ms (-1)=200) -> (element=w1511:T8, error out=w1519:errorcluster)  [unwired: 1 in, 2 out]
        n894 = Unbundle By Name(w1511) -> ("Action"=w1513:string)
        n895 = Empty String/Path?(string/path=w1513) -> (empty?=w1512:bool)
        n896 = case shown="False" w1512 {
          tunnel: w1515 -> [w1522 _]
          tunnel: w1511 -> [w1521 _]
          frame False {
            n897 = Generate User Event(user event=w1522, event data cluster=w1521) -> ()  [unwired: 2 in, 2 out]
          }
          frame True {
          }
        }
        n898 = Select(t="HALT;", s=w1519, f=w1516) -> (s? t:f=w1517:string)
      }
    }
  }
